vi "Consumer.vi"(8 "error in (no error)":errorcluster, 9 "Data":variant, 10 "Case ID":string, 11 "Tamer in":refnum<class "Tamer.lvclass">) -> (0 "error out":errorcluster, 3 "Tamer out":refnum<class "Tamer.lvclass">)   [LabVIEW 2020, in "Tamer.lvlib" / "Tamer.lvclass"]
uses:
  Tamer.lvclass
  C:/LabVIEW Code/CIRCUS/TALOS/TALOS_PPL.lvlibp/Ancestor/Ancestor/Ancestor.lvclass
  C:/LabVIEW Code/CIRCUS/TALOS/Actor Framework.lvlibp/1abvi3w/vi.lib/ActorFramework/Actor/Actor.lvclass
  C:/LabVIEW Code/CIRCUS/TALOS/TALOS_PPL.lvlibp/Father of all uServices/Father of all uServices/Father of all uServices.lvclass
  Tamer Consumer Case Selector.ctl
  Run Utilities/TypeDefs/Messages/Schedules With Sync Mask Message.ctl
  Run Utilities/Schedule/Schedule.lvclass
  Run Utilities/TypeDefs/Synchronize FPGA Cluster.ctl
  Tamer.lvclass/Tamer.ctl
  TALOS/TALOS_PPL.lvlibp/Ancestor/Ancestor/Infinite Message Selector.ctl
  TALOS/TALOS_PPL.lvlibp/Guardian/Guardian/Requests.ctl
  TALOS/TALOS_PPL.lvlibp/Support VIs/Go-NoGo.ctl
  Run Utilities/TypeDefs/Messages/Append Schedule Message.ctl
  Run Utilities/TypeDefs/Messages/Schedule Message.ctl
  Run Utilities/TypeDefs/DAQ Control.ctl
  Run Utilities/TypeDefs/Messages/Script Checker Message.ctl
  Run Utilities/TypeDefs/Script Checker Result.ctl
  Run Utilities/TypeDefs/Messages/Banana Message.ctl
  Run Utilities/TypeDefs/Return Code.ctl
  Internatl Banana.ctl
  Stop Message.ctl
  TALOS/Actor Framework.lvlibp/1abvi3w/vi.lib/ActorFramework/Message Enqueuer/Message Priority.ctl
  Run Utilities/TypeDefs/Messages/Monkey Status Message.ctl
  Run Utilities/TypeDefs/Monkey Status.ctl
  Monkey Summary.ctl
  Link Chain GUI.ctl
  TALOS/TALOS_PPL.lvlibp/Ancestor/Ancestor/Read ID.vi
  TALOS/TALOS_PPL.lvlibp/Support VIs/Global Constants.vi
  TALOS/TALOS_PPL.lvlibp/Father of all uServices/Father of all uServices/Children Methods/Get GUI Item Value - Variant.vi
  Tamer GV.vi
  TALOS/TALOS_PPL.lvlibp/Father of all uServices/Father of all uServices/Father of all uServices.lvclass
  Run Utilities/Run Utilities.lvlib
  TALOS/TALOS_PPL.lvlibp
  TALOS/TALOS_PPL.lvlibp/Guardian/Guardian/Guardian.lvclass
  TALOS/TALOS_PPL.lvlibp/Ancestor/Ancestor/Ancestor.lvclass
  C:/LabVIEW Code/CIRCUS/CIRCUS uServices et al/Tamer/Tamer.lvclass
  TALOS/TALOS_PPL.lvlibp/Guardian/Guardian Messages/Raise Abort Msg/Raise Abort Msg.lvclass
  TALOS/Actor Framework.lvlibp/1abvi3w/vi.lib/ActorFramework/Actor/Actor.lvclass
  TALOS/Actor Framework.lvlibp/1abvi3w/vi.lib/ActorFramework/Message Enqueuer/Message Enqueuer.lvclass
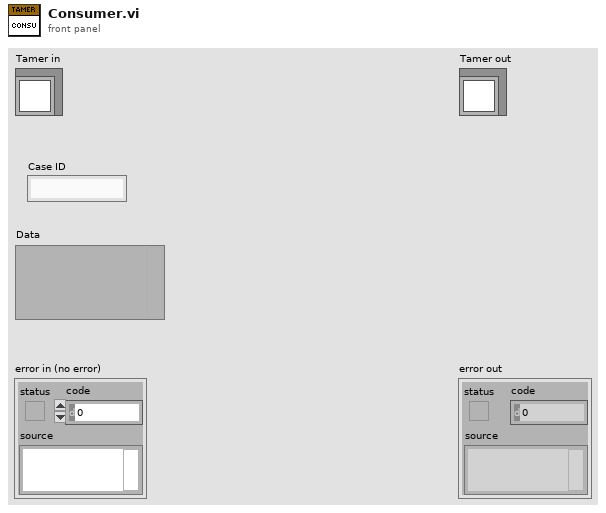
[diagram p1: front panel]
types:
  T1 = typedef "Tamer.lvlib/Tamer.lvclass/Tamer Consumer Case Selector.ctl" = enum16{"New schedule", "Initiate RUN", "Parse Schedules", "Script Checker", "Banana after Quality Check", "Update Crit Lvl", "Propagate Banana", "Reply from Guardian", "Reply from uService", "Timeout of RUN", "uService Replies Check", "Update from Monkey", "Monkey Died", "Reschedule", "Rerun", "Stop DAQ", "Stop Schedule", "Skip Run", "Kill Process", "Update GV", "Append"}
  T2 = typedef "Run Utilities.lvlib/Schedules With Sync Mask Message.ctl" = cluster{"Schedules":refnum<class "Schedule.lvclass">[], "Synchronised":T3[]}
  T3 = typedef "Run Utilities.lvlib/Synchronize FPGA Cluster.ctl" = cluster{"Status":bool, "FPGA Name":string}
  T4 = typedef "TALOS_PPL.lvlibp/Guardian.lvlib/Guardian.lvclass/Requests.ctl" = enum16{"Ready to Launch", "Start RUN", "Stop RUN", "Update DAQ Params", "Update Error Listbox", "Update Run Status", "Update Kasli Log", "Run Stopped with Errors", "Switch uS View"}
  T5 = typedef "TALOS_PPL.lvlibp/Go-NoGo.ctl" = cluster{"ID":string, "Status":bool, "Data":string[], "GUID":string}
  T6 = typedef "Run Utilities.lvlib/Append Schedule Message.ctl" = cluster{"List of FPGAs":set{string}, "Schedules":refnum<class "Schedule.lvclass">[], "To Top?":bool}
  T7 = typedef "Run Utilities.lvlib/Schedule Message.ctl" = cluster{"uS Name":string, "Synchronised":bool, "DAQ Control":T8, "Schedule":refnum<class "Schedule.lvclass">, "Append to top?":bool}
  T8 = typedef "Run Utilities.lvlib/DAQ Control.ctl" = enum16{"On", "Off", "External"}
  T9 = typedef "Run Utilities.lvlib/Script Checker Message.ctl" = cluster{"Monkey ID":string, "Script Checker Result":T10}
  T10 = typedef "Run Utilities.lvlib/Script Checker Result.ctl" = enum16{"Passed", "Failed", "Empty"}
  T11 = typedef "Run Utilities.lvlib/Banana Message.ctl" = cluster{"FPGA Name":string, "Return Code":T12}
  T12 = typedef "Run Utilities.lvlib/Return Code.ctl" = enum16{"All Good", "Retry", "Skip", "Skip All", "ABORT"}
  T13 = typedef "Tamer.lvlib/Tamer.lvclass/Internatl Banana.ctl" = cluster{"Process ID":string, "Return Code":T12}
  T14 = typedef "Tamer.lvlib/Tamer.lvclass/Stop Message.ctl" = cluster{"Gracefully":bool, "Process":string}
  T15 = typedef "Actor Framework.lvlibp/Message Enqueuer.lvclass/Message Priority.ctl" = enum16{"Low", "Normal", "High"}
  T16 = typedef "TALOS_PPL.lvlibp/Ancestor.lvlib/Ancestor.lvclass/Infinite Message Selector.ctl" = enum16{"Start", "Stop", "Check", "Flush (Stop all)", "Init"}
  T17 = typedef "Run Utilities.lvlib/Monkey Status Message.ctl" = cluster{"Monkey ID":string, "Monkey Status":T18, "Scripts left":u32, "ETA":string, "Current Action":string, "Report from previous RUNs":string, "Skipped RUNs":refnum<class "Schedule.lvclass">}
  T18 = typedef "Run Utilities.lvlib/Monkey Status.ctl" = enum16{"Init", "Paused", "Ongoing", "Stopped", "Finished (no errors)", "Finished (with errors)"}
  T19 = typedef "Tamer.lvlib/Tamer.lvclass/Monkey Summary.ctl" = cluster{"Color":u32, "Status":T18, "Continuous":bool, "Scripts left":u32, "Scripts skipped":u32, "ETA":string, "Current Action":string, "Report from previous RUNs":string, "Monkey ID":string, "With DAQ?":bool, "Linked?":T20, "Paused":bool}
  T20 = typedef "Tamer.lvlib/Tamer.lvclass/Link Chain GUI.ctl" = bool
  T21 = typedef "Tamer.lvlib/Tamer.lvclass/Tamer Status.ctl" = cluster{"Monkeys on the Stage":T19[], "All Monkeys Idle":bool}
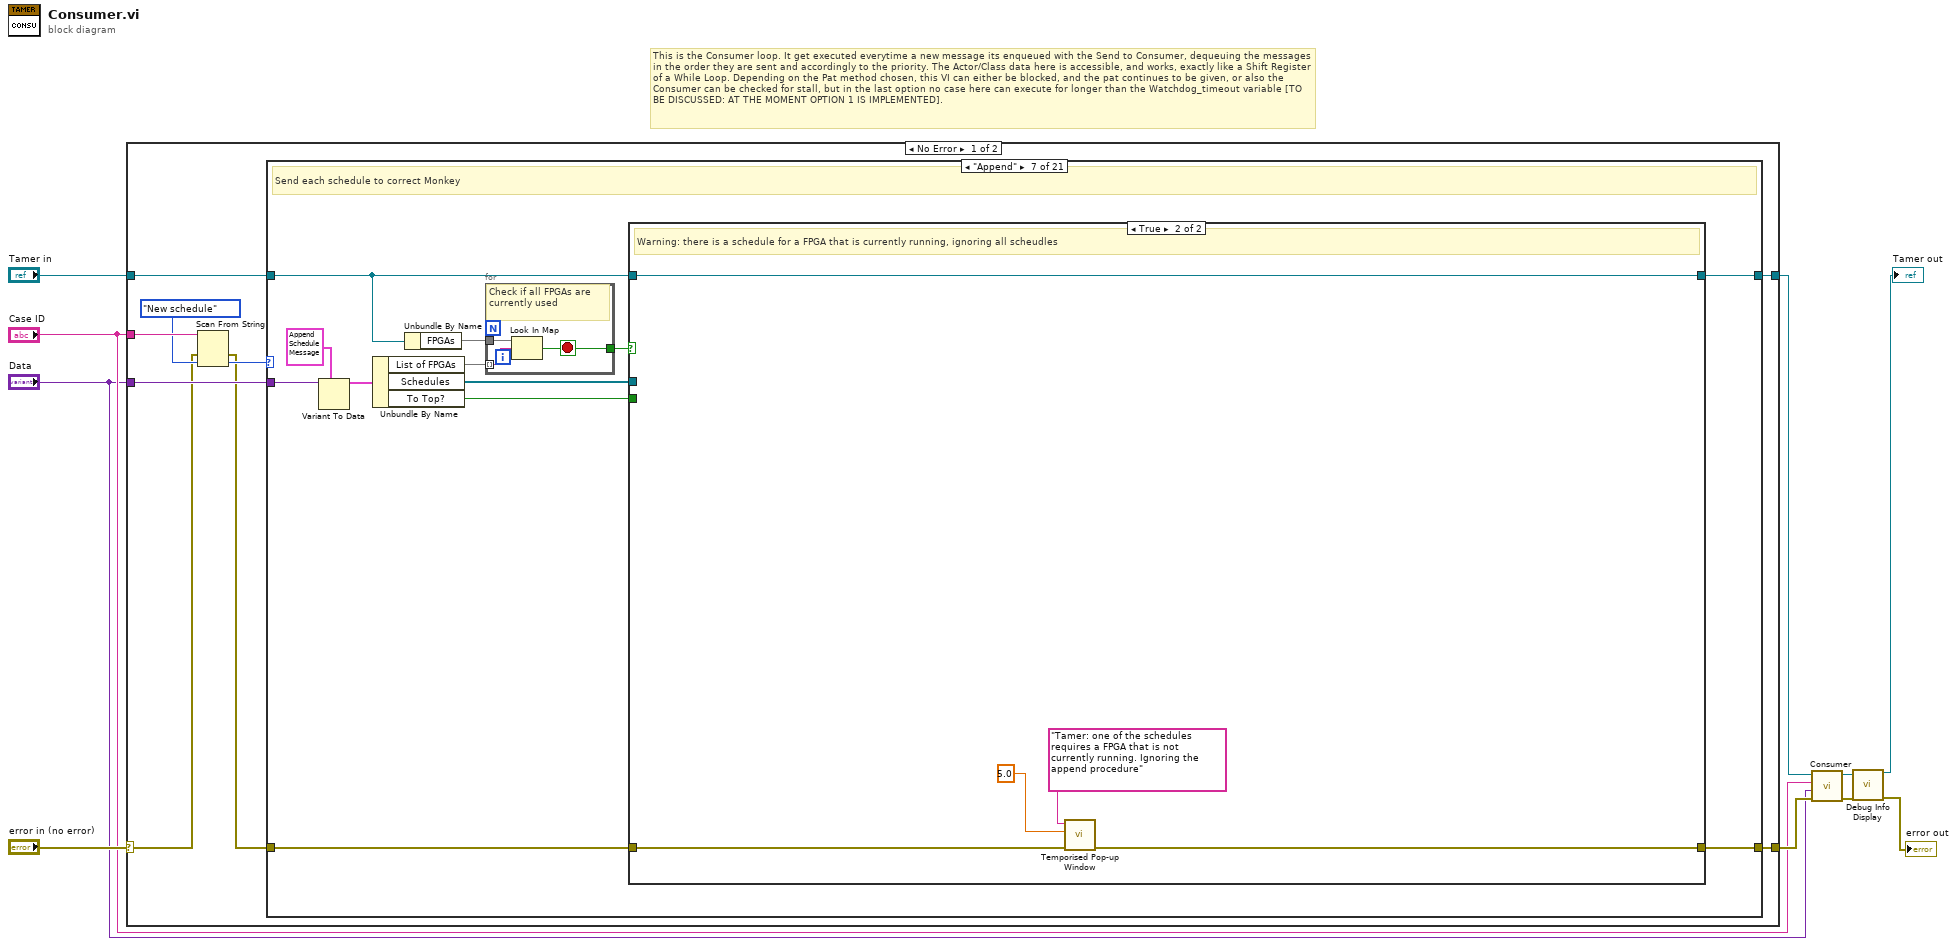
[diagram p0: block diagram]
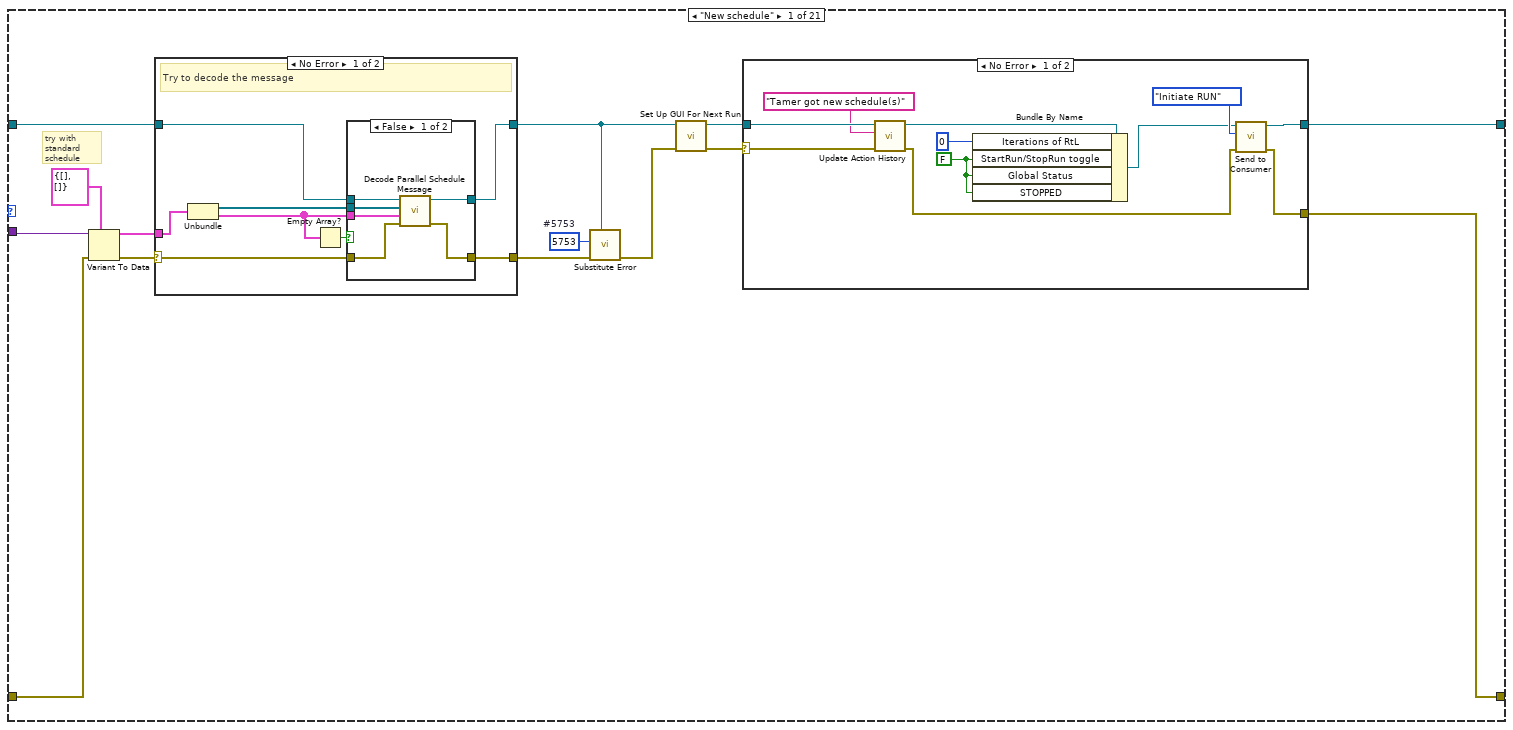
[diagram p2: hidden frame]
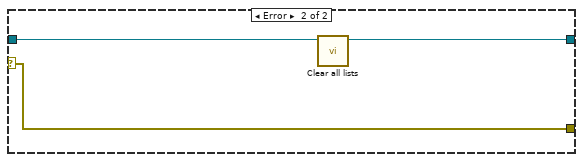
[diagram p3: hidden frame]
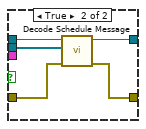
[diagram p4: hidden frame]
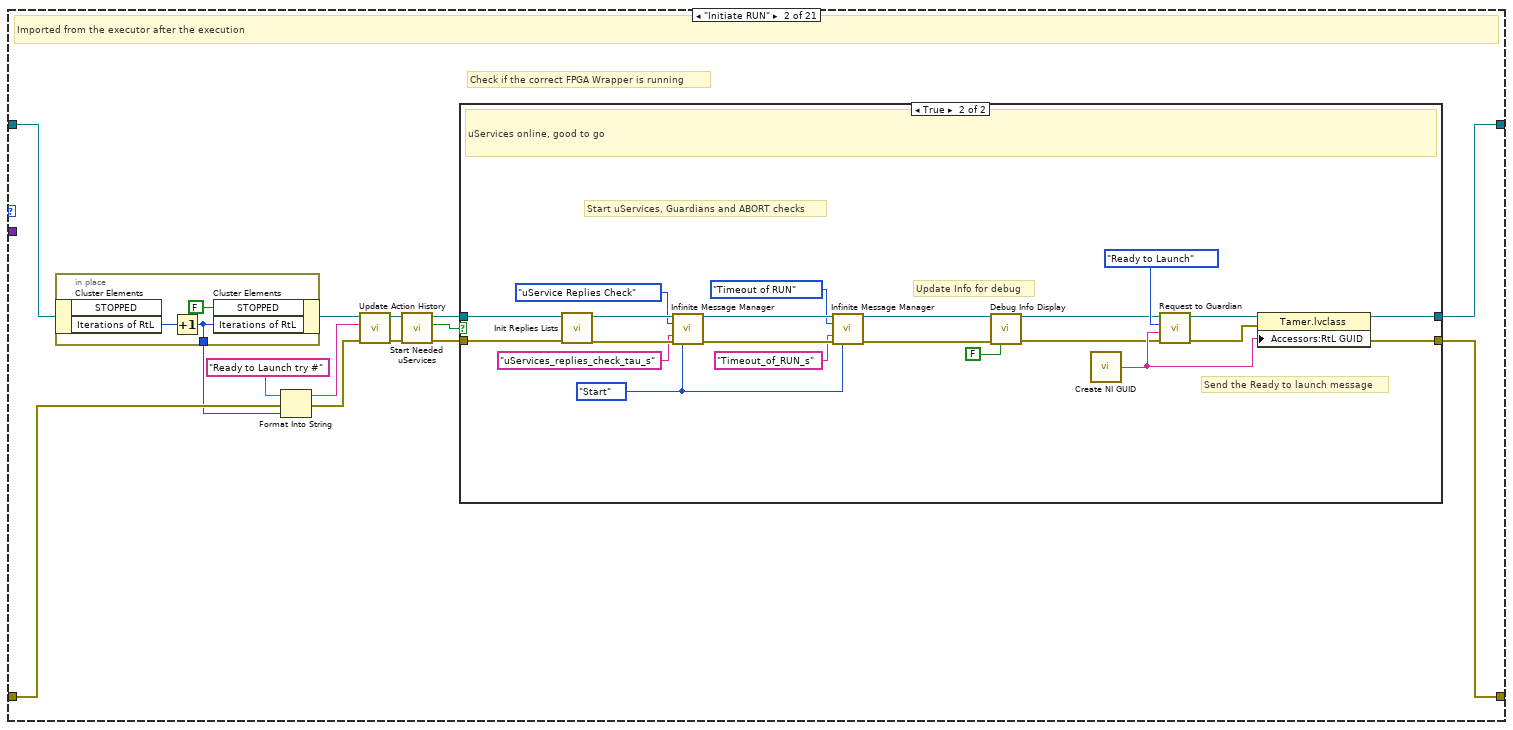
[diagram p6: hidden frame]
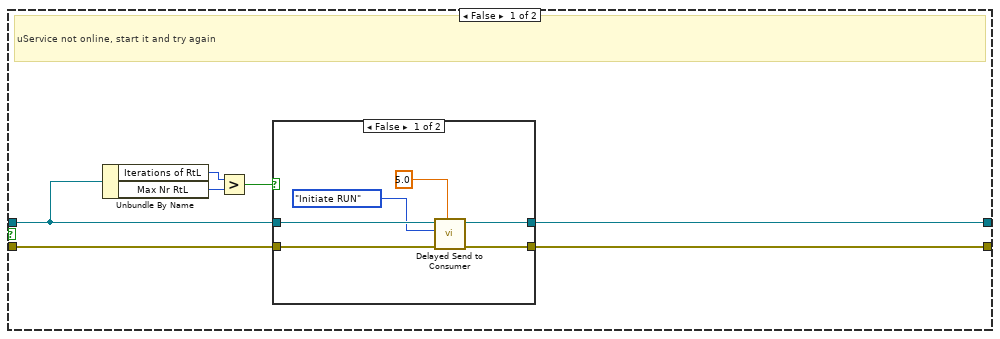
[diagram p7: hidden frame]
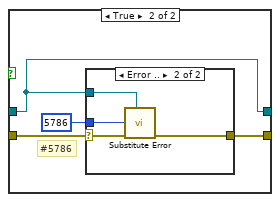
[diagram p8: hidden frame]
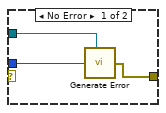
[diagram p9: hidden frame]
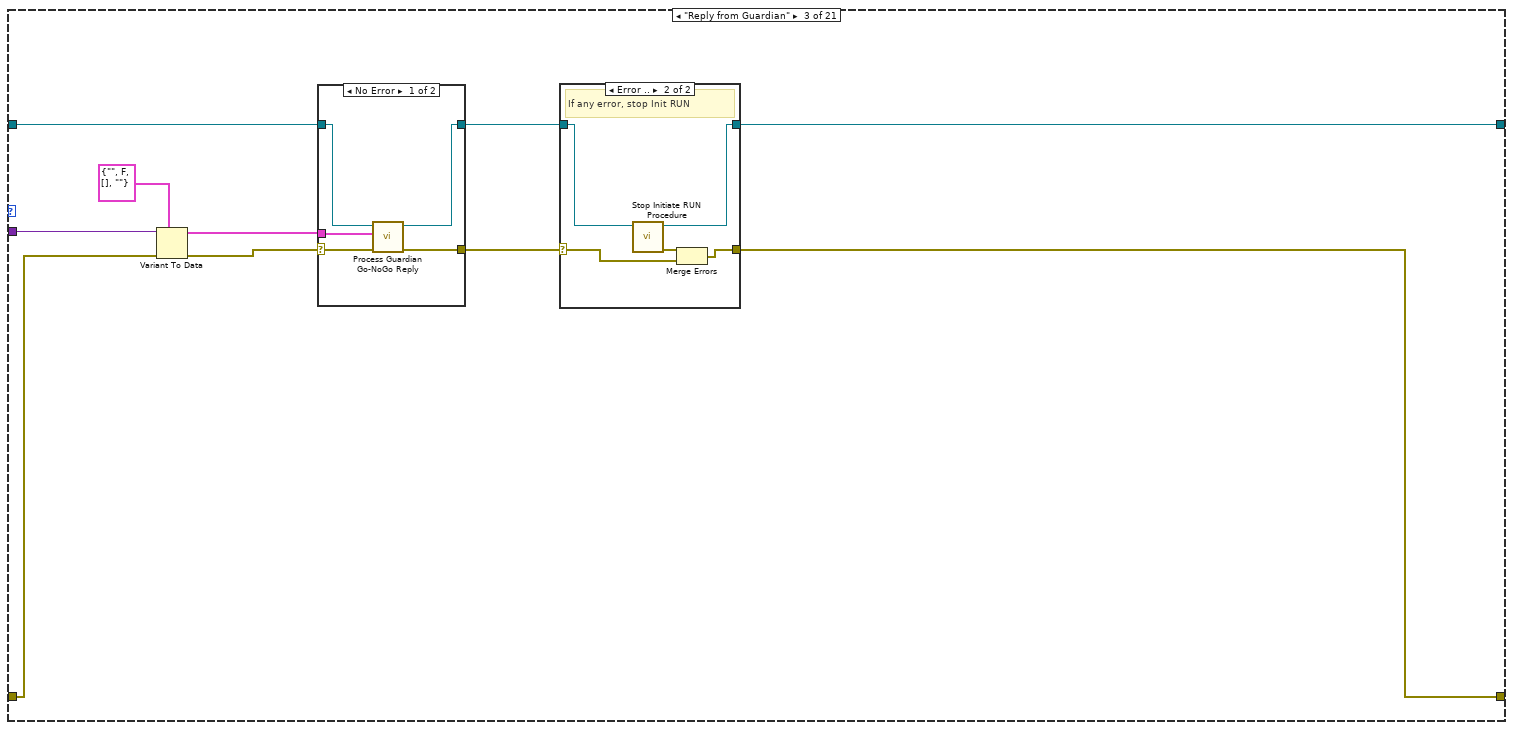
[diagram p10: hidden frame]
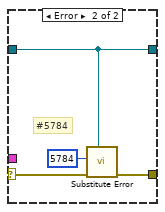
[diagram p12: hidden frame]
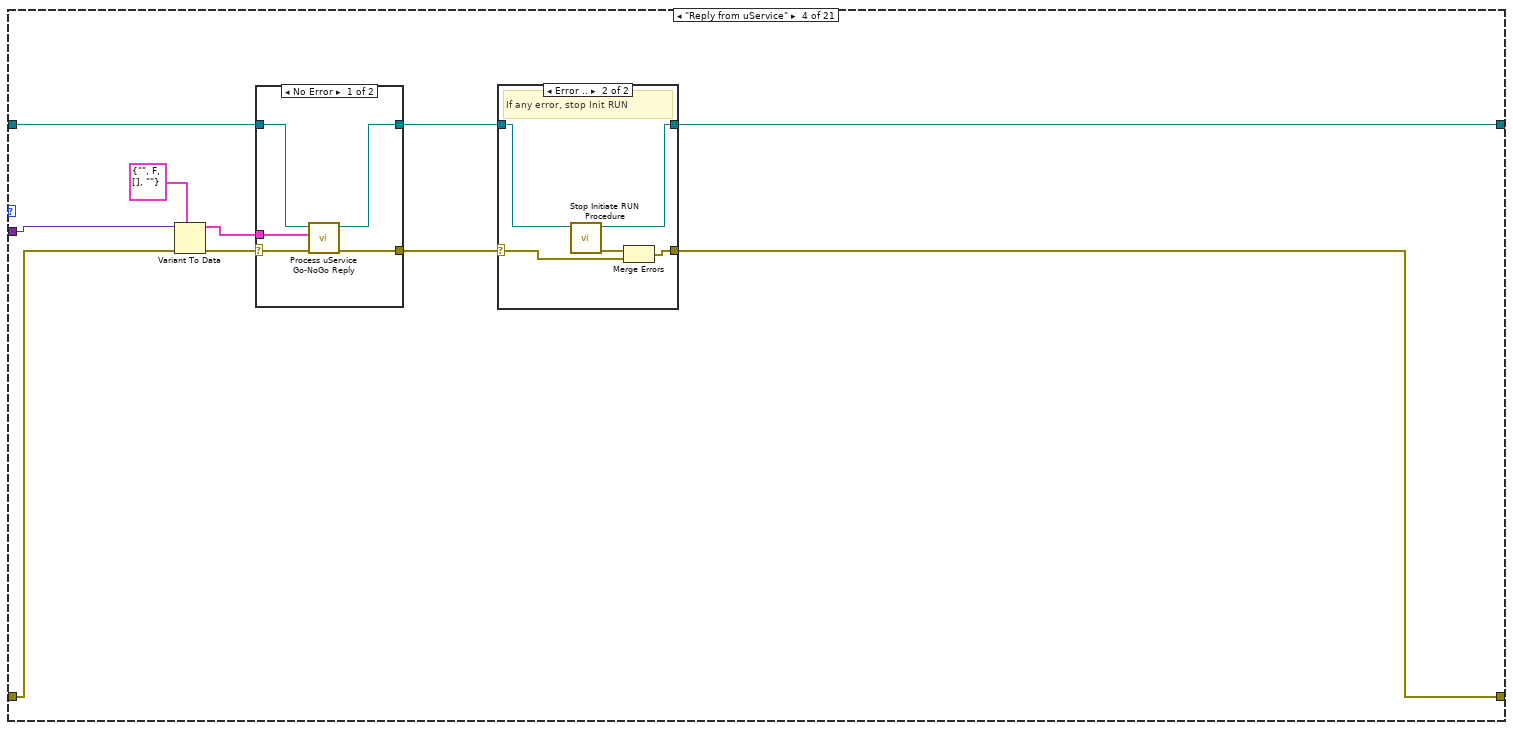
[diagram p13: hidden frame]
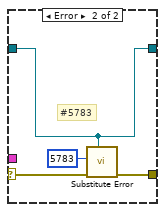
[diagram p15: hidden frame]
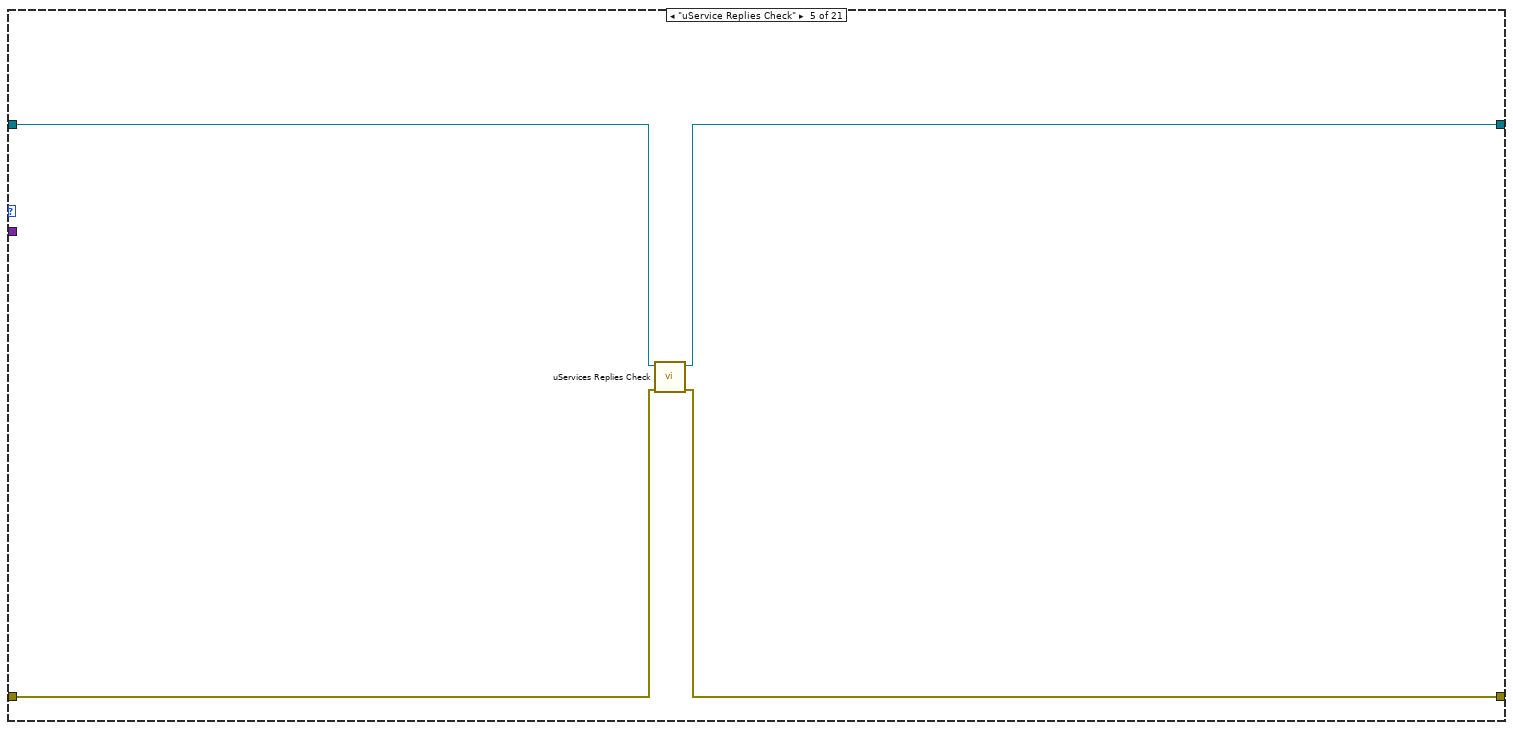
[diagram p16: hidden frame]
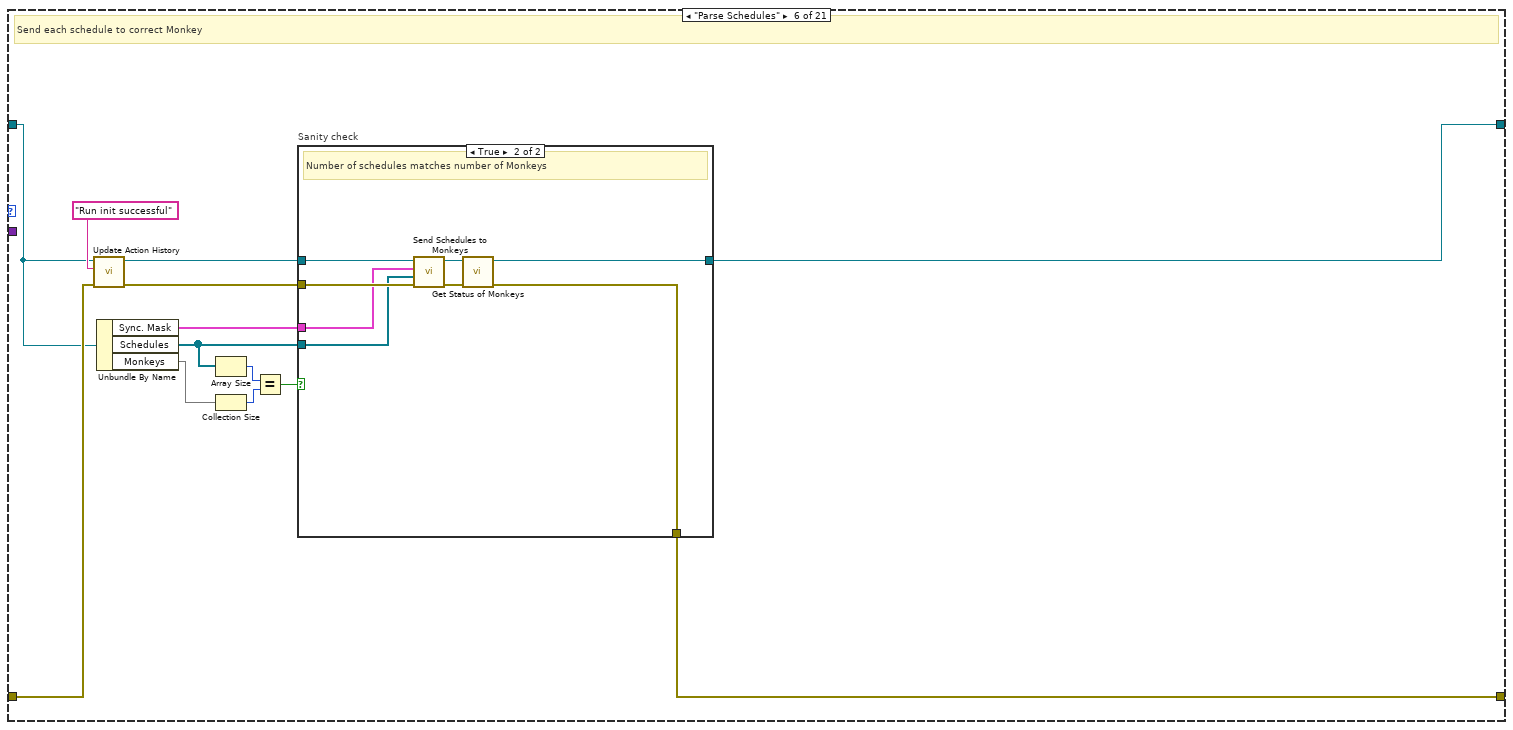
[diagram p17: hidden frame]
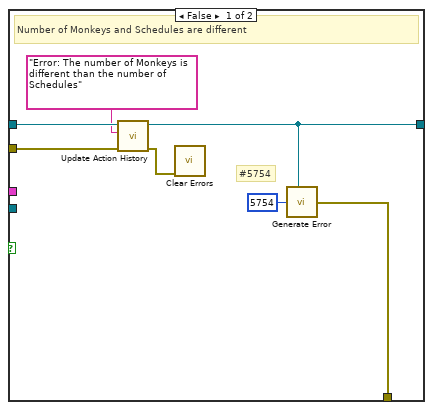
[diagram p18: hidden frame]
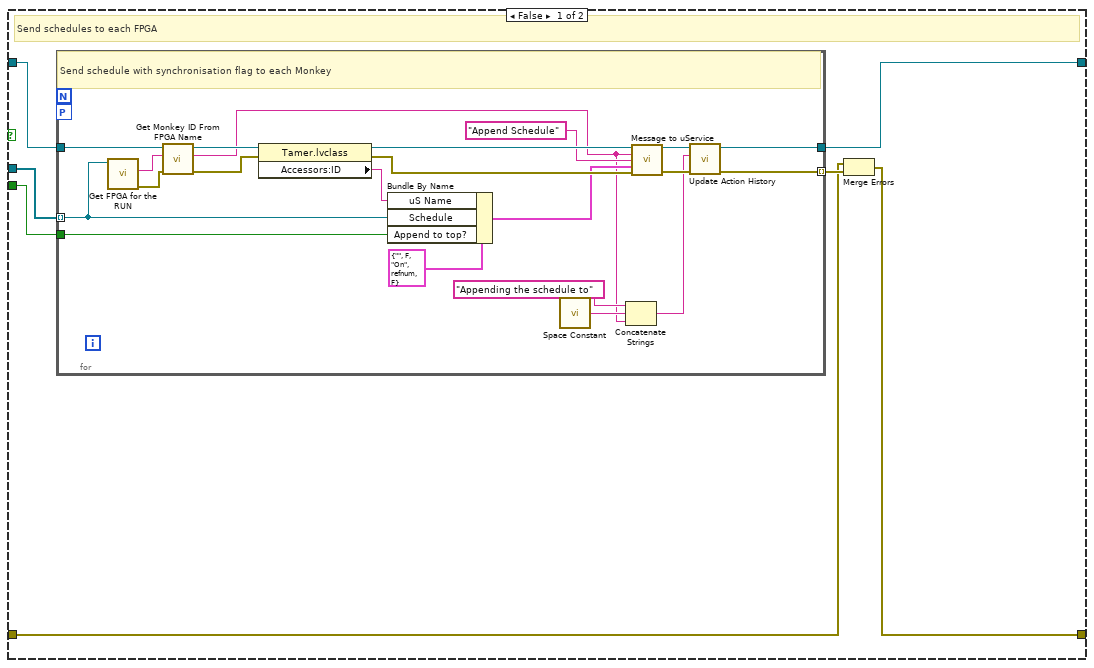
[diagram p19: hidden frame]
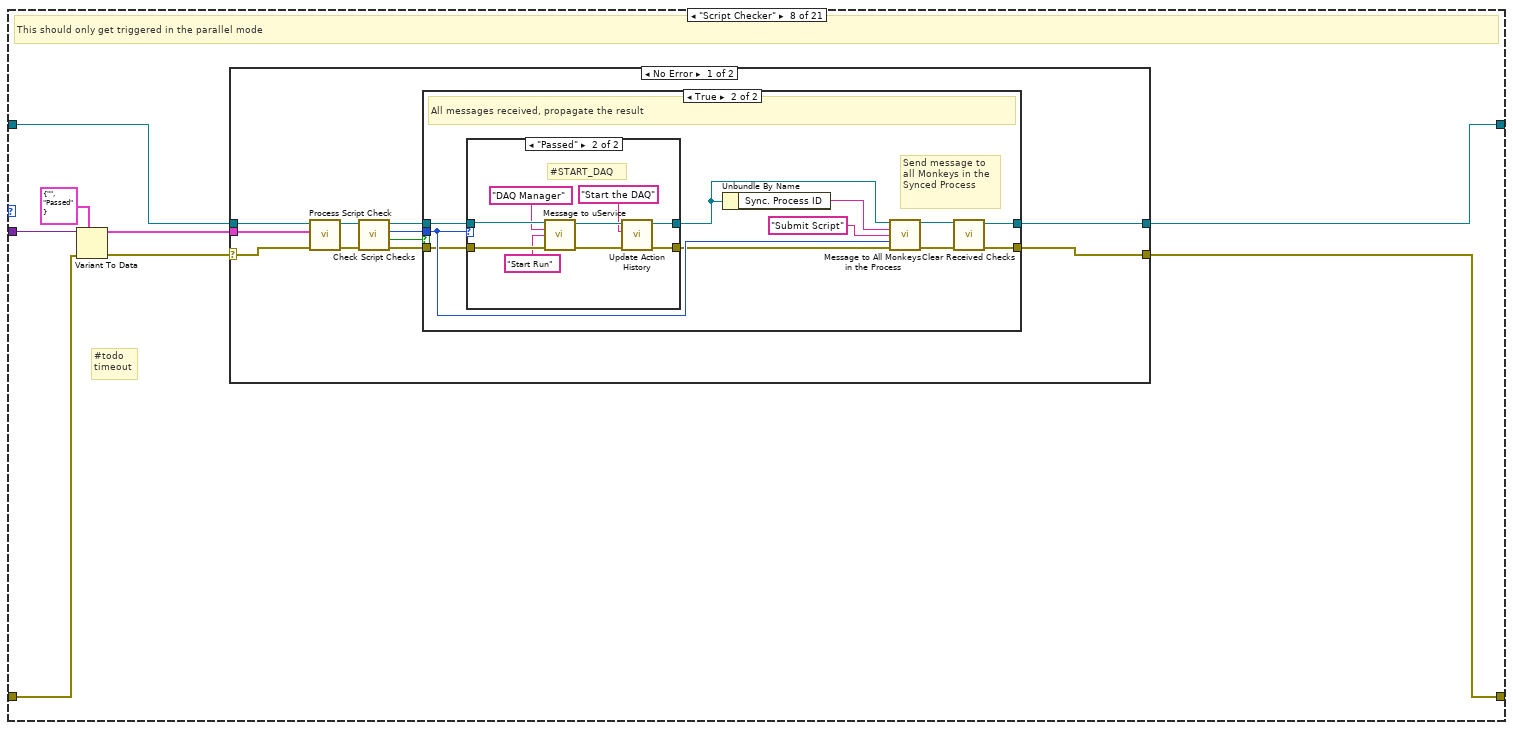
[diagram p20: hidden frame]
diagram:
  # "This is the Consumer loop. It get executed everytime a new message its enqueued with the Send to Consumer, dequeuing the messages in the order they are sent and accordingly to the priority. The Actor/Class data here is accessible, and works, exactly like a Shift Register of a While Loop. Depending on the Pat method chosen, this VI can either be blocked, and the pat continues to be given, or also the Consumer can be checked for stall, but in the last option no case here can execute for longer than the Watchdog_timeout variable [TO BE DISCUSSED: AT THE MOMENT OPTION 1 IS IMPLEMENTED]."
  n1 = case shown="No Error" "error in (no error)" {
    selector: "error in (no error)" -> [w12 w825]
    tunnel: [w18 w826] -> w7
    tunnel: "Tamer in" -> [w19 w826]
    tunnel: [w16 w825] -> w8
    tunnel: "Case ID" -> [w15 _]
    tunnel: "Data" -> [w17 _]
    frame No Error {
      n2 = Scan From String(input string=w15, error in=w12, default 1=Tamer_Consumer_Case_Selector."New schedule" ("Consumer Case Selector")) -> (error out=w11:errorcluster, output 1=w13:T1)  [unwired: 2 in, 2 out]
      n3 = case shown="\"Append\"" w13 {
        tunnel: w19 -> [w29 w69 w137 w163 w184 w191 w219 w266 w311 w378 w384 w403 w469 w485 w553 w593 w628 w677 w753 w817 w823]
        tunnel: [w26 w78 w136 w159 w185 w192 w218 w264 w318 w377 w386 w413 w466 w487 w552 w612 w634 w681 w755 w814 w820] -> w18
        tunnel: w17 -> [w31 _ w135 w162 _ _ w227 w271 w312 _ w390 w415 _ w490 w558 w599 w632 w682 w756 w813 _]
        tunnel: [w25 w77 w133 w160 w186 w198 w216 w265 w317 w375 w385 w412 w467 w486 w551 w611 w636 w680 w754 w815 w819] -> w16
        tunnel: w11 -> [w30 w82 w134 w161 w187 w195 w217 w269 w320 w376 w381 w414 w468 w488 w556 w600 w631 _ w757 w816 w822]
        frame "New schedule" {
          w23 = 5753  # #5753
          # "try with standard schedule"
          n4 = Variant To Data(error in=w30, type=T2 {"Schedules"=[], "Synchronised"=[]} ("Schedule message - parallel"), Variant=w31) -> (data=w32:T2, error out=w33:errorcluster)
          n5 = case shown="No Error" w33 {
            selector: w33 -> [w52 w67]
            tunnel: w32 -> [w48 _]
            tunnel: w29 -> [w54 w68]
            tunnel: [w53 w68] -> w20
            tunnel: [w51 w67] -> w22
            frame No Error {
              # "Try to decode the message"
              n6 = Unbundle(w48) -> ("Schedules"=w55:refnum<class "Schedule.lvclass">[], "Synchronised"=w50:T3[])
              n7 = Empty Array?(array=w50) -> (empty?=w49:bool)
              n8 = case shown="False" w49 {
                tunnel: w55 -> [w57 w66]
                tunnel: w54 -> [w58 w65]
                tunnel: [w59 w64] -> w53
                tunnel: w52 -> [w61 w63]
                tunnel: [w60 w62] -> w51
                tunnel: w50 -> [w56 _]
                frame False {
                  n9 = call-dynamic "Decode Parallel Schedule Message.vi"("error in (no error)"=w61, "Synchronised"=w56, "Schedules"=w57, "Tamer in"=w58) -> ("error out"=w60:errorcluster, "Tamer out"=w59:refnum<class "Tamer.lvclass">)  [unwired: 6 in]
                }
                frame True {
                  n10 = call-dynamic "Decode Schedule Message.vi"("error in (no error)"=w63, "Schedules"=w66, "Tamer in"=w65) -> ("error out"=w62:errorcluster, "Tamer out"=w64:refnum<class "Tamer.lvclass">)  [unwired: 7 in]
                }
              }
            }
            frame Error {
              # "Wrong message type from the Tamer"
            }
          }
          n11 = call "Substitute Error.vi"("LabVIEW Object"=w20, "error in (no error)"=w22, "Error Code"=w23) -> ("error out"=w21:errorcluster)  [unwired: 8 in]
          n12 = call-dynamic "Set Up GUI For Next Run.vi"("error in (no error)"=w21, "Tamer in"=w20) -> ("error out"=w27:errorcluster, "Tamer out"=w28:refnum<class "Tamer.lvclass">)  [unwired: 8 in]
          n13 = case shown="No Error" w27 {
            selector: w27 -> [w39 w47]
            tunnel: [w36 w45] -> w26
            tunnel: w28 -> [w44 w46]
            tunnel: [w34 w47] -> w25
            frame No Error {
              w40 = FALSE ("StartRun/StopRun toggle")
              n14 = call-dynamic "Update Action History.vi"("error in (no error)"=w39, "Action"="Tamer got new schedule(s)", "Tamer in"=w44) -> ("error out"=w35:errorcluster, "Tamer out"=w42:refnum<class "Tamer.lvclass">)  [unwired: 7 in]
              n15 = Bundle By Name(cluster=w42, "Iterations of RtL"=u8 0, "StartRun/StopRun toggle"=w40, "Global Status"=w40, "STOPPED"=w40) -> (w37:refnum<class "Tamer.lvclass">)
              n16 = call "Send to Consumer.vi"("error in (no error)"=w35, "Case ID"=Tamer_Consumer_Case_Selector."Initiate RUN" ("Monkey Consumer Case Selector"), "uService Template in"=w37) -> ("error out"=w34:errorcluster, "uService Template out"=w36:refnum<class "Tamer.lvclass">)  [unwired: 7 in]
            }
            frame Error {
              n17 = call-dynamic "Clear all lists.vi"("Tamer in"=w46) -> ("Tamer out"=w45:refnum<class "Tamer.lvclass">)  [unwired: 9 in, 1 out]
            }
          }
        }
        frame "Initiate RUN" {
          # "Check if the correct FPGA Wrapper is running"
          # "Imported from the executor after the execution"
          n18 = in-place {
            in-place-border: [w83] -> w70
            n19 = in-place-cluster #1(w69) -> ("Iterations of RtL"=w85:u8)  [unwired: 1 out]
            n20 = Increment(x=w85) -> (x+1=w83:u8)
            n21 = in-place-cluster #1("STOPPED"=FALSE, "Iterations of RtL"=w83) -> (w74:refnum<class "Tamer.lvclass">)
          }
          n22 = Format Into String(initial string="Ready to Launch try #", error in=w82, w70) -> (resulting string=w72:string, error out=w71:errorcluster)  [unwired: 1 in]
          n23 = call-dynamic "Update Action History.vi"("error in (no error)"=w71, "Action"=w72, "Tamer in"=w74) -> ("error out"=w75:errorcluster, "Tamer out"=w76:refnum<class "Tamer.lvclass">)  [unwired: 7 in]
          n24 = call-dynamic "Start Needed uServices.vi"("error in (no error)"=w75, "Tamer in"=w76) -> ("error out"=w80:errorcluster, "All online?"=w81:bool, "Tamer out"=w79:refnum<class "Tamer.lvclass">)  [unwired: 7 in]
          n25 = case shown="True" w81 {
            tunnel: w80 -> [w90 w113]
            tunnel: w79 -> [w89 w114]
            tunnel: [w92 w116] -> w78
            tunnel: [w91 w115] -> w77
            frame False {
              # "uService not online, start it and try again"
              n26 = Unbundle By Name(w89) -> ("Iterations of RtL"=w88:u8, "Max Nr RtL"=w87:u8)
              n27 = Greater?(x=w88, y=w87) -> (0:w86:bool)
              n28 = case shown="False" w86 {
                tunnel: [w98 w100] -> w92
                tunnel: [w97 w101] -> w91
                tunnel: w89 -> [w96 w100]
                tunnel: w90 -> [w95 w102]
                frame False {
                  n29 = call "Delayed Send to Consumer.vi"("Seconds (5)"=5.0 ("Delay"), "error in (no error)"=w95, "Case ID"=Tamer_Consumer_Case_Selector."Initiate RUN" ("Tamer Consumer Case Selector"), "Father of all uServices in"=w96) -> ("error out"=w97:errorcluster, "Father of all uServices out"=w98:refnum<class "Tamer.lvclass">)  [unwired: 6 in]
                }
                frame True {
                  # "#5786"
                  n30 = case shown="Error .." w102 {
                    selector: w102 -> [_ w109]
                    tunnel: [w103 w108] -> w101
                    tunnel: w100 -> [w105 w107]
                    tunnel: 5786 -> [w104 w106]
                    frame No Error {
                      n31 = call "Generate Error.vi"("Class"=w105, "Error Code"=w104) -> ("error out"=w103:errorcluster)  [unwired: 5 in]
                    }
                    frame Error {
                      n32 = call "Substitute Error.vi"("LabVIEW Object"=w107, "error in (no error)"=w109, "Error Code"=w106) -> ("error out"=w108:errorcluster)  [unwired: 8 in]
                    }
                  }
                }
              }
            }
            frame True {
              w124 = Infinite_Message_Selector."Start" ("Infinite Message Selector")
              # "Start uServices, Guardians and ABORT checks"
              # "Update Info for debug"
              # "Send the Ready to launch message"
              # "uServices online, good to go"
              n33 = call "Init Replies Lists.vi"("error in (no error)"=w113, "Monkey in"=w114) -> ("error out"=w128:errorcluster, "Monkey out"=w129:refnum<class "Tamer.lvclass">)  [unwired: 8 in]
              n34 = call-dynamic "Infinite Message Manager.vi"("Father of all uServices in"=w129, "Consumer Case Selector"=Tamer_Consumer_Case_Selector."uService Replies Check" ("Monkey Consumer Case Selector"), "Tau parameter"="uServices_replies_check_tau_s" ("SV Name"), "error in (no error)"=w128, "Infinite Message Selector"=w124) -> ("Father of all uServices out"=w126:refnum<class "Tamer.lvclass">, "error out"=w125:errorcluster)  [unwired: 8 in, 1 out]
              n35 = call-dynamic "Infinite Message Manager.vi"("Father of all uServices in"=w126, "Consumer Case Selector"=Tamer_Consumer_Case_Selector."Timeout of RUN" ("Monkey Consumer Case Selector"), "Tau parameter"="Timeout_of_RUN_s" ("SV Name"), "error in (no error)"=w125, "Infinite Message Selector"=w124) -> ("Father of all uServices out"=w120:refnum<class "Tamer.lvclass">, "error out"=w117:errorcluster)  [unwired: 8 in, 1 out]
              n36 = call-dynamic "Debug Info Display.vi"("Tamer in"=w120, "error in (no error)"=w117, "Do not clear"=FALSE) -> ("Tamer out"=w119:refnum<class "Tamer.lvclass">, "error out"=w118:errorcluster)  [unwired: 11 in]
              n37 = call <vilib>:"Create NI GUID.vi"() -> ("NI GUID"=w121:string)
              n38 = call "Request to Guardian.vi"("error in (no error)"=w118, "Data"=w121, "Requests"=Requests."Ready to Launch", "Father of all uServices in"=w119) -> ("error out"=w111:errorcluster, "Father of all uServices out"=w131:refnum<class "Tamer.lvclass">)  [unwired: 6 in]
              n39 = property class="Tamer.lvclass"(reference=w131, error in=w111, "Accessors:RtL GUID"=w121) -> (reference out=w116:refnum<class "Tamer.lvclass">, error out=w115:errorcluster)
            }
          }
        }
        frame "Reply from Guardian" {
          n40 = Variant To Data(error in=w134, type=T5 {"ID"="", "Status"=FALSE, "Data"=[], "GUID"=""} ("Go-NoGo"), Variant=w135) -> (data=w139:T5, error out=w140:errorcluster)
          n41 = case shown="No Error" w140 {
            selector: w140 -> [w153 w156]
            tunnel: [w152 w157] -> w141
            tunnel: w139 -> [w151 _]
            tunnel: w137 -> [w150 w154]
            tunnel: [w149 w154] -> w138
            frame No Error {
              n42 = call "Process Guardian Go-NoGo Reply.vi"("error in (no error)"=w153, "Go-NoGo"=w151, "Tamer in"=w150) -> ("error out"=w152:errorcluster, "Tamer out"=w149:refnum<class "Tamer.lvclass">)  [unwired: 7 in]
            }
            frame Error {
              # "#5784"
              n43 = call "Substitute Error.vi"("LabVIEW Object"=w154, "error in (no error)"=w156, "Error Code"=5784) -> ("error out"=w157:errorcluster)  [unwired: 8 in]
            }
          }
          n44 = case shown="Error .." w141 {
            selector: w141 -> [w143 w145]
            tunnel: [w143 w144] -> w133
            tunnel: [w142 w148] -> w136
            tunnel: w138 -> [w142 w147]
            frame No Error {
              # "All good!"
            }
            frame Error {
              # "If any error, stop Init RUN"
              n45 = call "Stop Initiate RUN Procedure.vi"("Tamer in"=w147) -> ("error out"=w146:errorcluster, "Tamer out"=w148:refnum<class "Tamer.lvclass">)  [unwired: 9 in]
              n46 = Merge Errors(w146, w145) -> (w144:errorcluster)
            }
          }
        }
        frame "Reply from uService" {
          n47 = Variant To Data(error in=w161, type=T5 {"ID"="", "Status"=FALSE, "Data"=[], "GUID"=""} ("Go-NoGo"), Variant=w162) -> (data=w167:T5, error out=w166:errorcluster)
          n48 = case shown="No Error" w166 {
            selector: w166 -> [w178 w182]
            tunnel: w167 -> [w179 _]
            tunnel: [w177 w183] -> w164
            tunnel: [w176 w180] -> w165
            tunnel: w163 -> [w175 w180]
            frame No Error {
              n49 = call "Process uService Go-NoGo Reply.vi"("error in (no error)"=w178, "Go-NoGo"=w179, "Tamer in"=w175) -> ("error out"=w177:errorcluster, "Tamer out"=w176:refnum<class "Tamer.lvclass">)  [unwired: 7 in]
            }
            frame Error {
              # "#5783"
              n50 = call "Substitute Error.vi"("LabVIEW Object"=w180, "error in (no error)"=w182, "Error Code"=5783) -> ("error out"=w183:errorcluster)  [unwired: 8 in]
            }
          }
          n51 = case shown="Error .." w164 {
            selector: w164 -> [w169 w170]
            tunnel: w165 -> [w168 w174]
            tunnel: [w169 w171] -> w160
            tunnel: [w168 w173] -> w159
            frame No Error {
              # "All good!"
            }
            frame Error {
              # "If any error, stop Init RUN"
              n52 = call "Stop Initiate RUN Procedure.vi"("Tamer in"=w174) -> ("error out"=w172:errorcluster, "Tamer out"=w173:refnum<class "Tamer.lvclass">)  [unwired: 9 in]
              n53 = Merge Errors(w172, w170) -> (w171:errorcluster)
            }
          }
        }
        frame "uService Replies Check" {
          n54 = call "uServices Replies Check.vi"("error in (no error)"=w187, "Tamer in"=w184) -> ("error out"=w186:errorcluster, "Tamer out"=w185:refnum<class "Tamer.lvclass">)  [unwired: 8 in]
        }
        frame "Parse Schedules" {
          # "Send each schedule to correct Monkey"
          n55 = call-dynamic "Update Action History.vi"("error in (no error)"=w195, "Action"="Run init successful", "Tamer in"=w191) -> ("error out"=w193:errorcluster, "Tamer out"=w196:refnum<class "Tamer.lvclass">)  [unwired: 7 in]
          n56 = Unbundle By Name(w191) -> ("Sync. Mask"=w200:T3[], "Schedules"=w199:refnum<class "Schedule.lvclass">[], "Monkeys"=w189:map{string, string[]})
          n57 = Array Size(array=w199) -> (size(s)=w190:i32)
          n58 = Collection Size(1:w189) -> (0:w188:i32)
          n59 = Equal?(x=w190, y=w188) -> (x = y?=w197:bool)
          n60 = case "Sanity check" shown="True" w197 {
            tunnel: w200 -> [_ w212]
            tunnel: w196 -> [w205 w214]
            tunnel: w199 -> [_ w213]
            tunnel: [w206 w208] -> w198
            tunnel: w193 -> [w204 w215]
            tunnel: [w201 w210] -> w192
            frame False {
              # "#5754"
              # "Number of Monkeys and Schedules are different"
              n61 = call-dynamic "Update Action History.vi"("error in (no error)"=w204, "Action"="Error: The number of Monkeys is different than the number of Schedules", "Tamer in"=w205) -> ("error out"=w202:errorcluster, "Tamer out"=w201:refnum<class "Tamer.lvclass">)  [unwired: 7 in]
              n62 = call <vilib>:"Clear Errors.vi"("error in (no error)"=w202) -> ()  [unwired: 5 in, 2 out]
              n63 = call "Generate Error.vi"("Class"=w201, "Error Code"=5754) -> ("error out"=w206:errorcluster)  [unwired: 5 in]
            }
            frame True {
              # "Number of schedules matches number of Monkeys"
              n64 = call "Send Schedules to Monkeys.vi"("error in (no error)"=w215, "Schedules"=w213, "Sync. Mask"=w212, "Tamer in"=w214) -> ("error out"=w209:errorcluster, "Tamer out"=w211:refnum<class "Tamer.lvclass">)  [unwired: 6 in]
              n65 = call-dynamic "Get Status of Monkeys.vi"("error in (no error)"=w209, "Tamer in"=w211) -> ("error out"=w208:errorcluster, "Tamer out"=w210:refnum<class "Tamer.lvclass">)  [unwired: 7 in, 1 out]
            }
          }
        }
        frame "Append" {
          # "Send each schedule to correct Monkey"
          n66 = Variant To Data(type=T6 {"List of FPGAs"={}, "Schedules"=[], "To Top?"=FALSE} ("Schedule message"), Variant=w227) -> (data=w225:T6)  [unwired: 1 in, 1 out]
          n67 = Unbundle By Name(w225) -> ("List of FPGAs"=w224:set{string}, "Schedules"=w221:refnum<class "Schedule.lvclass">[], "To Top?"=w220:bool)
          n68 = Unbundle By Name(w219) -> ("FPGAs"=w223:map{string, string})
          n69 = for {
            tunnel: w224 -> [w262] mode=indexing
            tunnel: w223 -> [w263]
            tunnel: [w261] -> w222
            stop <- w261 stop-if-true
            # "Check if all FPGAs are currently used"
            n70 = Look In Map(map=w263, key=w262) -> (key not found?=w261:bool)  [unwired: 1 in, 1 out]
          }
          n71 = case shown="True" w222 {
            tunnel: w221 -> [w232 _]
            tunnel: w220 -> [w231 _]
            tunnel: w219 -> [w234 w260]
            tunnel: [w233 w260] -> w218
            tunnel: w217 -> [w228 w257]
            tunnel: [w229 w256] -> w216
            frame False {
              # "Send schedules to each FPGA"
              n72 = for {
                tunnel: w234 -> [w244]
                tunnel: w232 -> [w238] mode=indexing
                tunnel: [w236] -> w230 mode=indexing
                tunnel: [w237] -> w233
                workers-P: _ -> [_]
                tunnel: w231 -> [w235]
                # "Send schedule with synchronisation flag to each Monkey"
                n73 = call-dynamic "Get FPGA for the RUN.vi"("Schedule in"=w238) -> ("error out"=w241:errorcluster, "FPGA Name"=w242:string)  [unwired: 8 in, 1 out]
                n74 = call-dynamic "Get Monkey ID From FPGA Name.vi"("error in (no error)"=w241, "FPGA Name"=w242, "Tamer in"=w244) -> ("error out"=w240:errorcluster, "Monkey ID"=w239:string, "Tamer out"=w243:refnum<class "Tamer.lvclass">)  [unwired: 6 in]
                n75 = property class="Tamer.lvclass"(reference=w243, error in=w240) -> (reference out=w252:refnum<class "Tamer.lvclass">, error out=w255:errorcluster, "Accessors:ID"=w251:string)
                n76 = Bundle By Name(cluster=T7 {"uS Name"="", "Synchronised"=FALSE, "DAQ Control"=enum."On", "Schedule"=refnum, "Append to top?"=FALSE} ("Monkey Schedule Message"), "uS Name"=w251, "Schedule"=w238, "Append to top?"=w235) -> (w254:T7)
                n77 = call <vilib>:"Space Constant.vi"() -> ("String"=w246:string)
                n78 = Concatenate Strings("Appending the schedule to" ("string"), w246, w239) -> (w248:string)
                n79 = call "Message to uService.vi"("Father of all uServices in"=w252, "uService ID"=w239, "Message"="Append Schedule", "Data"=w254, "error in (no error)"=w255) -> ("Father of all uServices out"=w250:refnum<class "Tamer.lvclass">, "error out"=w249:errorcluster)  [unwired: 9 in]
                n80 = call-dynamic "Update Action History.vi"("error in (no error)"=w249, "Action"=w248, "Tamer in"=w250) -> ("error out"=w236:errorcluster, "Tamer out"=w237:refnum<class "Tamer.lvclass">)  [unwired: 7 in]
              }
              n81 = Merge Errors(w228, w230) -> (w229:errorcluster)
            }
            frame True {
              # "Warning: there is a schedule for a FPGA that is currently running, ignoring all scheudles"
              n82 = call "Temporised Pop-up Window.vi"("error in (no error)"=w257, "Timeout"=5.0, "Text"="Tamer: one of the schedules requires a FPGA that is not currently running. Ignoring the append procedure") -> ("error out"=w256:errorcluster)  [unwired: 8 in]
            }
          }
        }
        frame "Script Checker" {
          # "#todo\ntimeout"
          # "This should only get triggered in the parallel mode"
          n83 = Variant To Data(error in=w269, type=T9 {"Monkey ID"="", "Script Checker Result"=enum."Passed"} ("Message"), Variant=w271) -> (data=w267:T9, error out=w268:errorcluster)
          n84 = case shown="No Error" w268 {
            selector: w268 -> [w282 w310]
            tunnel: w267 -> [w273 _]
            tunnel: w266 -> [w274 w308]
            tunnel: [w272 w309] -> w265
            tunnel: [w275 w308] -> w264
            frame No Error {
              n85 = call-dynamic "Process Script Check.vi"("error in (no error)"=w282, "Message"=w273, "Tamer in"=w274) -> ("error out"=w280:errorcluster, "Tamer out"=w281:refnum<class "Tamer.lvclass">)  [unwired: 7 in]
              n86 = call-dynamic "Check Script Checks.vi"("error in (no error)"=w280, "Tamer in"=w281) -> ("error out"=w278:errorcluster, "Send Result?"=w279:bool, "Script Checker Result"=w277:T10, "Tamer out"=w276:refnum<class "Tamer.lvclass">)  [unwired: 6 in]
              n87 = case shown="True" w279 {
                tunnel: w278 -> [w283 w288]
                tunnel: w277 -> [_ w293]
                tunnel: w276 -> [w284 w287]
                tunnel: [w283 w290] -> w272
                tunnel: [w284 w289] -> w275
                frame False {
                  # "Waiting for some responses"
                }
                frame True {
                  # "Send message to all Monkeys in the Synced Process"
                  # "All messages received, propagate the result"
                  n88 = case shown="\"Passed\"" w293 {
                    tunnel: w287 -> [w297 w300]
                    tunnel: w288 -> [w296 w303]
                    tunnel: [w296 w302] -> w285
                    tunnel: [w297 w301] -> w286
                    frame Default {
                    }
                    frame "Passed" {
                      # "#START_DAQ"
                      n89 = call "Message to uService.vi"("Father of all uServices in"=w300, "uService ID"="DAQ Manager", "Message"="Start Run", "error in (no error)"=w303) -> ("Father of all uServices out"=w305:refnum<class "Tamer.lvclass">, "error out"=w306:errorcluster)  [unwired: 10 in]
                      n90 = call-dynamic "Update Action History.vi"("error in (no error)"=w306, "Action"="Start the DAQ", "Tamer in"=w305) -> ("error out"=w302:errorcluster, "Tamer out"=w301:refnum<class "Tamer.lvclass">)  [unwired: 7 in]
                    }
                  }
                  n91 = Unbundle By Name(w286) -> ("Sync. Process ID"=w294:string)
                  n92 = call-dynamic "Message to All Monkeys in the Process.vi"("Tamer in"=w286, "Process ID"=w294, "Message"="Submit Script", "Data"=w293, "error in (no error)"=w285) -> ("Tamer out"=w292:refnum<class "Tamer.lvclass">, "error out"=w291:errorcluster)  [unwired: 9 in]
                  n93 = call-dynamic "Clear Received Checks.vi"("error in (no error)"=w291, "Tamer in"=w292) -> ("error out"=w290:errorcluster, "Tamer out"=w289:refnum<class "Tamer.lvclass">)  [unwired: 8 in]
                }
              }
            }
            frame Error {
              # "#5207"
              n94 = call "Substitute Error.vi"("LabVIEW Object"=w308, "error in (no error)"=w310, "Error Code"=5207) -> ("error out"=w309:errorcluster)  [unwired: 8 in]
            }
          }
        }
        frame "Banana after Quality Check" {
          # "This case is needed to avoid the race condition of an error getting enqueued immediately after the Run is finished: the Monkey would then skip the Criticality Level associated to that error (and, by the way, using it in the subsequent Run). In this way, the \"What to do next\" will be enqued after any - reasonably - possible \"Error Criticality\" message from the Error Manager."
          n95 = Variant To Data(error in=w320, type=T11 {"FPGA Name"="", "Return Code"=enum."All Good"} ("Cluster"), Variant=w312) -> (data=w315:T11, error out=w316:errorcluster)
          n96 = case shown="Error .." w316 {
            selector: w316 -> [w321 _]
            tunnel: w315 -> [w322 _]
            tunnel: [w322 w331] -> w314
            tunnel: [w321 w327] -> w313
            tunnel: w312 -> [_ w330]
            tunnel: w311 -> [_ w326]
            frame No Error {
            }
            frame Error {
              n97 = Variant To Data(type="", Variant=w330) -> (data=w325:string, error out=w328:errorcluster)  [unwired: 1 in]
              n98 = call-dynamic "Get FPGA Name From Monkey ID.vi"("error in (no error)"=w328, "Monkey ID"=w325, "Tamer in"=w326) -> ("error out"=w327:errorcluster, "FPGA Name"=w324:string)  [unwired: 6 in, 1 out]
              n99 = Bundle By Name(cluster=T11 {"FPGA Name"="", "Return Code"=enum."All Good"} ("Cluster"), "Return Code"=Return_Code."Skip", "FPGA Name"=w324) -> (w331:T11)
            }
          }
          n100 = case shown="No Error" w313 {
            selector: w313 -> [w340 w369]
            tunnel: [w336 w373] -> w318
            tunnel: [w333 w372] -> w317
            tunnel: w311 -> [w335 w373]
            tunnel: w314 -> [w334 _]
            frame No Error {
              n101 = call-dynamic "Process Banana Message.vi"("error in (no error)"=w340, "Message"=w334, "Tamer in"=w335) -> ("error out"=w341:errorcluster, "Propagate Banana?"=w339:bool, "Internal Banana"=w337:T13, "Tamer out"=w338:refnum<class "Tamer.lvclass">)  [unwired: 5 in]
              n102 = case shown="True" w339 {
                tunnel: w338 -> [w343 w353]
                tunnel: w341 -> [w342 w354]
                tunnel: w337 -> [_ w344]
                tunnel: [w343 w348] -> w336
                tunnel: [w342 w346] -> w333
                frame False {
                  # "Do not propagate Banana (maybe not all Monkeys finished, or there was ABORT)"
                }
                frame True {
                  # "avoid enqueuing a new script before the previous one has finished"
                  # "Let's Propagate with a delay"
                  n103 = Unbundle By Name(w353) -> ("Sync. Process ID"=w352:string)
                  n104 = Unbundle By Name(w344) -> ("Process ID"=w351:string)
                  n105 = Equal?(x=w352, y=w351) -> (x = y?=w350:bool)
                  n106 = case shown="True" w350 {
                    tunnel: w354 -> [w358 w367]
                    tunnel: [w361 w368] -> w349
                    tunnel: [w356 w367] -> w347
                    tunnel: w353 -> [w360 w368]
                    tunnel: [w362 1.0] -> w355
                    frame True {
                      # "#STOP_DAQ"
                      # "In synchronised we need to stop DAQ"
                      n107 = call "Send to Consumer.vi"("error in (no error)"=w358, "Case ID"=Tamer_Consumer_Case_Selector."Stop DAQ" ("Consumer Case Selector"), "uService Template in"=w360) -> ("error out"=w357:errorcluster, "uService Template out"=w361:refnum<class "Tamer.lvclass">)  [unwired: 7 in]
                      n108 = call "TALOS Config Param.vi"("error in (no error)"=w357, "Parameter Name"="Stop_DAQ_Delay_s") -> ("error out"=w356:errorcluster, "Output"=w364:string)  [unwired: 8 in]
                      n109 = Fract/Exp String To Number(string=w364, default (0 dbl)=10.0 ("default (0 DBL)")) -> (number=w362:dbl)  [unwired: 2 in, 1 out]
                    }
                    frame False {
                      # "Not synchronised, just send it"
                    }
                  }
                  n110 = call "Delayed Send to Consumer.vi"("Seconds (5)"=w355, "error in (no error)"=w347, "Data"=w344, "Case ID"=Tamer_Consumer_Case_Selector."Propagate Banana" ("Consumer Case Selector"), "Father of all uServices in"=w349) -> ("error out"=w346:errorcluster, "Father of all uServices out"=w348:refnum<class "Tamer.lvclass">)  [unwired: 5 in]
                }
              }
            }
            frame Error {
              # "#5207"
              n111 = call "Substitute Error.vi"("LabVIEW Object"=w373, "error in (no error)"=w369, "Error Code"=5207, "Optional String"="Wrong banana message!") -> ("error out"=w372:errorcluster)  [unwired: 7 in]
            }
          }
        }
        frame "Stop DAQ" {
          # "#STOP_DAQ"
          n112 = call "Message to uService.vi"("Father of all uServices in"=w378, "uService ID"="DAQ Manager", "Message"="Stop Run", "error in (no error)"=w376) -> ("Father of all uServices out"=w377:refnum<class "Tamer.lvclass">, "error out"=w375:errorcluster)  [unwired: 10 in]
        }
        frame "Propagate Banana" {
          # "By default, I mean"
          # "#Stop or ABORT?"
          # "Send Processed Banana to each Monkey that needs to receive it"
          n113 = call-dynamic "Update Action History.vi"("error in (no error)"=w381, "Action"="Propagate Banana", "Tamer in"=w384) -> ("error out"=w382:errorcluster, "Tamer out"=w383:refnum<class "Tamer.lvclass">)  [unwired: 7 in]
          n114 = Variant To Data(error in=w382, type=T13 {"Process ID"="", "Return Code"=enum."All Good"} ("Internal Banana"), Variant=w390) -> (data=w388:T13, error out=w387:errorcluster)
          n115 = case shown="No Error" w387 {
            selector: w387 -> [w395 w402]
            tunnel: w388 -> [w398 _]
            tunnel: [w394 w400] -> w386
            tunnel: [w393 w401] -> w385
            tunnel: w383 -> [w391 w400]
            frame No Error {
              n116 = Unbundle By Name(w398) -> ("Process ID"=w397:string, "Return Code"=w396:T12)
              n117 = call-dynamic "Message to All Monkeys in the Process.vi"("Tamer in"=w391, "Process ID"=w397, "Message"="B4N4N4", "Data"=w396, "error in (no error)"=w395) -> ("Tamer out"=w394:refnum<class "Tamer.lvclass">, "error out"=w393:errorcluster)  [unwired: 9 in]
            }
            frame Error {
              # "#5207"
              n118 = call "Substitute Error.vi"("LabVIEW Object"=w400, "error in (no error)"=w402, "Error Code"=5207) -> ("error out"=w401:errorcluster)  [unwired: 8 in]
            }
          }
        }
        frame "Update Crit Lvl" {
          # "Volpe: it is correct to forward the criticality level to each Monkey and let them handle it, because if they are running async, they need to independently choose what to do"
          # "If there was an error in variant to data, it means that the variant was empty: no specific error was provided. Ignore that error"
          # "Send Criticality level to every Running Monkey. so it knows"
          n119 = Variant To Data(error in=w414, type=u8 0, Variant=w415) -> (data=w410:u8, error out=w411:errorcluster)
          n120 = global read "Global Constants.vi" "ABORT Crt Lvl"() -> (w406:u8)
          n121 = case shown="No Error" w411 {
            selector: w411 -> [w459 w464]
            tunnel: w410 -> [w460 _]
            tunnel: [w460 w461] -> w409
            tunnel: [w459 w463] -> w408
            tunnel: w406 -> [_ w462]
            frame No Error {
            }
            frame Error {
              n122 = call <vilib>:"Clear Errors.vi"("error in (no error)"=w464) -> ("error out"=w463:errorcluster)  [unwired: 5 in, 1 out]
              n123 = Decrement(x=w462) -> (x-1=w461:u8)
            }
          }
          n124 = case shown="No Error" w408 {
            selector: w408 -> [w444 w458]
            tunnel: w409 -> [w447 _]
            tunnel: [w443 w457] -> w405
            tunnel: [w442 w455] -> w404
            tunnel: w406 -> [w441 w455]
            tunnel: w403 -> [w440 w454]
            frame No Error {
              n125 = In Range and Coerce(upper limit=w441, x=w447, lower limit=u8 0) -> (In Range?=w445:bool)  [unwired: 1 out]
              n126 = case shown="False" w445 {
                tunnel: w447 -> [_ w453]
                tunnel: w444 -> [_ w452]
                tunnel: [w451 w452] -> w443
                tunnel: [w449 w453] -> w442
                tunnel: w441 -> [w449 _]
                tunnel: w440 -> [w448 _]
                frame False {
                  # "#5788"
                  n127 = call "Generate Error.vi"("Class"=w448, "Error Code"=5788) -> ("error out"=w451:errorcluster)  [unwired: 5 in]
                }
                frame True {
                  # "All good!"
                }
              }
            }
            frame Error {
              # "#5788"
              n128 = call "Substitute Error.vi"("LabVIEW Object"=w454, "error in (no error)"=w458, "Error Code"=5788) -> ("error out"=w457:errorcluster)  [unwired: 8 in]
            }
          }
          n129 = case shown="4" w404 {
            selector: w404 -> [w416 _ _]
            tunnel: w403 -> [w420 w431 w436]
            tunnel: w405 -> [w419 w429 w433]
            tunnel: [w417 w423 w438] -> w413
            tunnel: [w418 w428 w432] -> w412
            frame Default {
              n130 = call-dynamic "Send Error Criticality.vi"("error in (no error)"=w419, "Crit. Level"=w416, "Tamer in"=w420) -> ("error out"=w418:errorcluster, "Tamer out"=w417:refnum<class "Tamer.lvclass">)  [unwired: 5 in]
            }
            frame 3 {
              # "To stop gracefully all the running processes"
              n131 = call "Send to Consumer.vi"("Data"=T14 {"Gracefully"=TRUE, "Process"="ALL"} ("cluster"), "Case ID"=Tamer_Consumer_Case_Selector."Stop Schedule" ("Monkey Consumer Case Selector"), "uService Template in"=w431) -> ("error out"=w424:errorcluster, "uService Template out"=w425:refnum<class "Tamer.lvclass">)  [unwired: 7 in]
              n132 = call "Request to Guardian.vi"("error in (no error)"=w424, "Data"=FALSE, "Requests"=Requests."Run Stopped with Errors", "Father of all uServices in"=w425) -> ("error out"=w422:errorcluster, "Father of all uServices out"=w423:refnum<class "Tamer.lvclass">)  [unwired: 6 in]
              n133 = Merge Errors(w422, w429) -> (w428:errorcluster)
            }
            frame 4 {
              # "Let safe mode do the work"
              n134 = call "Read Caller Enqueuer.vi"("Actor"=w436) -> ("Caller Enqueuer"=w435:refnum<class "Message Enqueuer.lvclass">)  [unwired: 10 in]
              n135 = call "Send Raise Abort.vi"("Message Priority (Normal)"=Message_Priority."High", "error in (no error)"=w433, "Message Enqueuer"=w435) -> ("error out"=w432:errorcluster)  [unwired: 7 in, 1 out]
              n136 = call "Request to Guardian.vi"("Data"=FALSE, "Requests"=Requests."Run Stopped with Errors", "Father of all uServices in"=w436) -> ("Father of all uServices out"=w438:refnum<class "Tamer.lvclass">)  [unwired: 7 in, 1 out]
            }
          }
        }
        frame "Timeout of RUN" {
          # "Checks if someone has already stopped Timeout of RUN (but this message has already get enqueued): in case, do nothing, because it means that the RUN Init Procedure has completed successfully (albeit just in time). In case Timeout of RUN was still on, terminate the RUN Init Procedure and thow the timeout error."
          # "Stop the RUN Init Procedure and raise ABORT."
          n137 = call-dynamic "Infinite Message Manager.vi"("Father of all uServices in"=w469, "Consumer Case Selector"=Tamer_Consumer_Case_Selector."Timeout of RUN" ("Monkey Consumer Case Selector"), "Infinite Message Selector"=Infinite_Message_Selector."Check") -> ("Father of all uServices out"=w473:refnum<class "Tamer.lvclass">, "Exists?"=w472:bool, "error out"=w471:errorcluster)  [unwired: 10 in]
          n138 = case shown="True" w472 {
            tunnel: [w476 w482] -> w466
            tunnel: w473 -> [w476 w477]
            tunnel: [w475 w481] -> w474
            tunnel: w471 -> [w475 w479]
            frame False {
            }
            frame True {
              # "#5778"
              n139 = call "Substitute Error.vi"("LabVIEW Object"=w477, "error in (no error)"=w479, "Error Code"=5778) -> ("error out"=w478:errorcluster)  [unwired: 8 in]
              n140 = call "Stop Initiate RUN Procedure.vi"("error in (no error)"=w478, "Tamer in"=w477) -> ("error out"=w481:errorcluster, "Tamer out"=w482:refnum<class "Tamer.lvclass">)  [unwired: 8 in]
            }
          }
          n141 = Merge Errors(w474, w468) -> (w467:errorcluster)
        }
        frame "Update from Monkey" {
          n142 = Variant To Data(error in=w488, type=T17 {"Monkey ID"="", "Monkey Status"=enum."Init", "Scripts left"=0, "ETA"="", "Current Action"="", "Report from previous RUNs"="", "Skipped RUNs"=refnum} ("Monkey Status Message"), Variant=w490) -> (data=w483:T17, error out=w484:errorcluster)
          n143 = case shown="No Error" w484 {
            selector: w484 -> [w500 w550]
            tunnel: [w493 w548] -> w487
            tunnel: [w492 w549] -> w486
            tunnel: w485 -> [w501 w548]
            tunnel: w483 -> [w499 _]
            frame No Error {
              n144 = Unbundle By Name(w499) -> ("Monkey ID"=w496:string, "Monkey Status"=w491:T18)
              n145 = call-dynamic "Process Monkey Report.vi"("error in (no error)"=w500, "Monkey Status Message"=w499, "Tamer in"=w501) -> ("error out"=w504:errorcluster, "Tamer out"=w505:refnum<class "Tamer.lvclass">)  [unwired: 7 in]
              n146 = Concatenate Strings("Received update from " ("string"), w496) -> (w498:string)
              n147 = call-dynamic "Update Action History.vi"("error in (no error)"=w504, "Action"=w498, "Tamer in"=w505) -> ("error out"=w502:errorcluster, "Tamer out"=w503:refnum<class "Tamer.lvclass">)  [unwired: 7 in]
              n148 = call-dynamic "Get Status of Monkeys.vi"("error in (no error)"=w502, "Tamer in"=w503) -> ("error out"=w506:errorcluster, "Anything running?"=w508:bool, "Tamer out"=w507:refnum<class "Tamer.lvclass">)  [unwired: 7 in]
              n149 = case shown="False" w508 {
                tunnel: w507 -> [w528 w541]
                tunnel: w506 -> [w527 w543]
                tunnel: [w518 w544] -> w495
                tunnel: [w517 w542] -> w494
                tunnel: w496 -> [w526 _]
                frame False {
                  n150 = Unbundle By Name(w528) -> ("STOPPED"=w529:bool)
                  n151 = case shown="True" w529 {
                    tunnel: w528 -> [w533 w540]
                    tunnel: w527 -> [w532 w539]
                    tunnel: [w533 w540] -> w523
                    tunnel: [w532 w539] -> w520
                    tunnel: w526 -> [_ w535]
                    tunnel: [w530 w534] -> w519
                    frame False {
                      w530 = "All Monkeys Finished" ("Action")
                      n152 = call "Temporised Pop-up Window.vi"("error in (no error)"=w532, "Timeout"=5.0, "Text"=w530) -> ()  [unwired: 8 in, 1 out]
                    }
                    frame True {
                      n153 = call <vilib>:"Space Constant.vi"() -> ("String"=w538:string)
                      n154 = Concatenate Strings("STOPPED:" ("string"), w535, w538, " Finished" ("Action")) -> (w534:string)
                    }
                  }
                  n155 = call "Request to Guardian.vi"("error in (no error)"=w520, "Data"=FALSE, "Requests"=Requests."Update Run Status", "Father of all uServices in"=w523) -> ("error out"=w521:errorcluster, "Father of all uServices out"=w522:refnum<class "Tamer.lvclass">)  [unwired: 6 in]
                  n156 = call-dynamic "Update Action History.vi"("error in (no error)"=w521, "Action"=w519, "Tamer in"=w522) -> ("error out"=w517:errorcluster, "Tamer out"=w518:refnum<class "Tamer.lvclass">)  [unwired: 7 in]
                }
                frame True {
                  n157 = call "Request to Guardian.vi"("error in (no error)"=w543, "Data"=TRUE, "Requests"=Requests."Update Run Status", "Father of all uServices in"=w541) -> ("error out"=w542:errorcluster, "Father of all uServices out"=w544:refnum<class "Tamer.lvclass">)  [unwired: 6 in]
                }
              }
              n158 = case shown="\"Finished (with errors)\"" w491 {
                tunnel: w495 -> [w510 w514]
                tunnel: w494 -> [w509 w513]
                tunnel: [w510 w512] -> w493
                tunnel: [w509 w511] -> w492
                frame Default {
                }
                frame "Finished (with errors)" {
                  n159 = call "Request to Guardian.vi"("error in (no error)"=w513, "Data"=FALSE, "Requests"=Requests."Run Stopped with Errors", "Father of all uServices in"=w514) -> ("error out"=w511:errorcluster, "Father of all uServices out"=w512:refnum<class "Tamer.lvclass">)  [unwired: 6 in]
                }
              }
            }
            frame Error {
              # "#5207"
              n160 = call "Substitute Error.vi"("LabVIEW Object"=w548, "error in (no error)"=w550, "Error Code"=5207) -> ("error out"=w549:errorcluster)  [unwired: 8 in]
            }
          }
        }
        frame "Monkey Died" {
          n161 = Variant To Data(error in=w556, type="" ("Monkey ID"), Variant=w558) -> (data=w554:string, error out=w555:errorcluster)
          n162 = case shown="No Error" w555 {
            selector: w555 -> [w570 w587]
            tunnel: w554 -> [w567 _]
            tunnel: w553 -> [w576 w588]
            tunnel: [w559 w588] -> w552
            tunnel: [w560 w586] -> w551
            frame No Error {
              w564 = "The Stage" ("FP Item Name")
              n163 = call-poly "Get GUI Item Value.vi"("FP Item Name"=w564, "uService Template in"=w576) -> ("error out"=w575:errorcluster, "Value"=w574:variant)  [unwired: 7 in, 1 out]
              n164 = Unbundle By Name(w576) -> ("Monkeys"=w572:map{string, string[]})
              n165 = Variant To Data(error in=w575, type=T19[][] [] ("2D Synchronous Monkeys"), Variant=w574) -> (data=w569:T19[][])  [unwired: 1 out]
              n166 = Collection Size(1:w572) -> (0:w571:i32)
              n167 = call "Cast 2D to 1D.vi"("1D size"=w571, "2D Synchronous Monkeys"=w569) -> ("1D Synchronous Monkeys"=w568:T19[])
              n168 = call-dynamic "Monkey Died.vi"("error in (no error)"=w570, "Monkey ID"=w567, "Tamer in"=w576) -> ("error out"=w562:errorcluster, "Tamer out"=w563:refnum<class "Tamer.lvclass">)  [unwired: 7 in]
              n169 = for {
                tunnel: w568 -> [w584] mode=indexing
                tunnel: w567 -> [w583]
                tunnel: [w584] -> w566 mode=indexing if=w578
                # "Remove the Monkey from the GUI"
                n170 = Unbundle By Name(w584) -> ("Monkey ID"=w582:string)
                n171 = Empty String/Path?(string/path=w582) -> (empty?=w581:bool)
                n172 = Not Equal?(x=w582, y=w583) -> (x != y?=w579:bool)
                n173 = Not(x=w581) -> (.not. x?=w580:bool)
                n174 = And(x=w580, y=w579) -> (x .and. y?=w578:bool)
              }
              n175 = call-dynamic "Update Process Indicator.vi"("error in (no error)"=w562, "Tamer in"=w563) -> ("error out"=w561:errorcluster, "Tamer out"=w577:refnum<class "Tamer.lvclass">)  [unwired: 8 in]
              n176 = call "Cast 1D to 2D.vi"("1D Monkeys"=w566) -> ("2D Monkeys"=w565:T19[][])
              n177 = call "Update GUI.vi"("error in (no error)"=w561, "Data"=w565, "GUI Item Name"=w564, "uService Template in"=w577) -> ("error out"=w560:errorcluster, "uService Template out"=w559:refnum<class "Tamer.lvclass">)  [unwired: 6 in]
            }
            frame Error {
              # "#5773"
              n178 = call "Substitute Error.vi"("LabVIEW Object"=w588, "error in (no error)"=w587, "Error Code"=5773) -> ("error out"=w586:errorcluster)  [unwired: 8 in]
            }
          }
        }
        frame "Reschedule" {
          w598 = ""  # Process ID
          # "#5775"
          n179 = Variant To Data(error in=w600, type=w598, Variant=w599) -> (data=w589:string, error out=w597:errorcluster)
          n180 = case shown="\"ALL\"" w589 {
            selector: w589 -> [_ w618]
            tunnel: w593 -> [w616 w622]
            tunnel: w597 -> [w614 w621]
            tunnel: [w616 w620] -> w601
            tunnel: [w615 w617] -> w603
            tunnel: [w614 w619] -> w602
            frame "ALL" {
              n181 = Unbundle By Name(w616) -> ("Schedules"=w615:refnum<class "Schedule.lvclass">[])  [unwired: 1 out]
            }
            frame Default {
              n182 = call-dynamic "Get Schedules for the Process.vi"("error in (no error)"=w621, "Process ID"=w618, "Tamer in"=w622) -> ("error out"=w619:errorcluster, "Schedules"=w617:refnum<class "Schedule.lvclass">[], "Tamer out"=w620:refnum<class "Tamer.lvclass">)  [unwired: 5 in, 1 out]
            }
          }
          n183 = call "Message to uService.vi"("Father of all uServices in"=w601, "uService ID"="Scheduler" ("string"), "Message"="Reschedule", "Data"=w603, "error in (no error)"=w602) -> ("Father of all uServices out"=w592:refnum<class "Tamer.lvclass">, "error out"=w590:errorcluster)  [unwired: 9 in]
          n184 = call-dynamic "Get List of Monkeys in the Process.vi"("error in (no error)"=w590, "Process ID"=w589, "Tamer in"=w592) -> ("error out"=w613:errorcluster, "List of Monkeys"=w596:string[], "Tamer out"=w591:refnum<class "Tamer.lvclass">)  [unwired: 5 in, 1 out]
          n185 = call <vilib>:"Space Constant.vi"() -> ("String"=w608:string)
          n186 = call <vilib>:"1D String Array to Delimited String.vi"("delimiter"=", ", "string array"=w596) -> ("delimited string"=w594:string)  [unwired: 9 in]
          n187 = Concatenate Strings("Sending the schedule(s) from" ("string"), w608, w594) -> (w607:string)
          n188 = call-dynamic "Update Action History.vi"("error in (no error)"=w613, "Action"=w607, "Tamer in"=w591) -> ("error out"=w610:errorcluster, "Tamer out"=w612:refnum<class "Tamer.lvclass">)  [unwired: 7 in]
          n189 = call "Substitute Error.vi"("LabVIEW Object"=w612, "error in (no error)"=w610, "Error Code"=5775, "Optional String"=w594) -> ("error out"=w611:errorcluster)  [unwired: 7 in]
        }
        frame "Rerun" {
          w630 = ""  # Process ID
          # "#5774"
          n190 = Variant To Data(error in=w631, type=w630, Variant=w632) -> (data=w626:string, error out=w629:errorcluster)
          n191 = call-dynamic "Get Status of Monkeys.vi"("Tamer in"=w628) -> ("Anything running?"=w624:bool, "Tamer out"=w627:refnum<class "Tamer.lvclass">)  [unwired: 8 in, 1 out]
          n192 = Empty String/Path?(string/path=w626) -> (empty?=w625:bool)
          n193 = Or(x=w624, y=w625) -> (x .or. y?=w623:bool)
          n194 = case shown="False" w623 {
            tunnel: [w641 w676] -> w634
            tunnel: [w640 w675] -> w633
            tunnel: w629 -> [w639 w675]
            tunnel: w627 -> [w638 w676]
            tunnel: w626 -> [w637 _]
            frame False {
              n195 = case "Update Monkey status" shown="\"ALL\"" w637 {
                selector: w637 -> [w644 _]
                tunnel: [w653 w671] -> w641
                tunnel: [w651 w670] -> w640
                tunnel: w639 -> [w642 w667]
                tunnel: w638 -> [w643 w664]
                frame Default {
                  # "Update status of Monkeys in the proces"
                  n196 = call-dynamic "Get Schedules for the Process.vi"("error in (no error)"=w642, "Process ID"=w644, "Tamer in"=w643) -> ("error out"=w647:errorcluster, "Schedules"=w646:refnum<class "Schedule.lvclass">[], "Sync. Mask"=w645:T3[], "Tamer out"=w648:refnum<class "Tamer.lvclass">)  [unwired: 5 in]
                  n197 = call "Send Schedules to Monkeys.vi"("error in (no error)"=w647, "Schedules"=w646, "Sync. Mask"=w645, "Tamer in"=w648) -> ("error out"=w649:errorcluster, "Tamer out"=w650:refnum<class "Tamer.lvclass">)  [unwired: 6 in]
                  n198 = call-dynamic "Get List of Monkeys in the Process.vi"("error in (no error)"=w649, "Process ID"=w644, "Tamer in"=w650) -> ("error out"=w654:errorcluster, "List of Monkeys"=w655:string[], "Tamer out"=w656:refnum<class "Tamer.lvclass">)  [unwired: 5 in, 1 out]
                  n199 = for {
                    tunnel: w655 -> [w660] mode=indexing
                    tunnel: w654 -> [w661]
                    shift-right: [w659] -> w653
                    shift-left: w656 -> [w662]
                    tunnel: [w658] -> w652 mode=indexing
                    n200 = call-dynamic "Update Monkeys Status.vi"("Overwrite"=TRUE, "error in (no error)"=w661, "Status"=Monkey_Status."Init", "Monkey ID"=w660, "Tamer in"=w662) -> ("error out"=w658:errorcluster, "Tamer out"=w659:refnum<class "Tamer.lvclass">)  [unwired: 5 in]
                  }
                  n201 = Merge Errors(w652) -> (w651:errorcluster)
                }
                frame "ALL" {
                  # "Update status of all the Monkeys"
                  n202 = Unbundle By Name(w664) -> ("Sync. Mask"=w665:T3[], "Schedules"=w666:refnum<class "Schedule.lvclass">[])
                  n203 = call "Send Schedules to Monkeys.vi"("error in (no error)"=w667, "Schedules"=w666, "Sync. Mask"=w665, "Tamer in"=w664) -> ("error out"=w674:errorcluster, "Tamer out"=w668:refnum<class "Tamer.lvclass">)  [unwired: 6 in]
                  n204 = call-dynamic "Update Monkeys Status.vi"("Overwrite"=TRUE, "In ALL?"=TRUE, "error in (no error)"=w674, "Status"=Monkey_Status."Init", "Tamer in"=w668) -> ("error out"=w670:errorcluster, "Tamer out"=w671:refnum<class "Tamer.lvclass">)  [unwired: 5 in]
                }
              }
            }
            frame True {
            }
          }
          n205 = call "Substitute Error.vi"("LabVIEW Object"=w634, "error in (no error)"=w633, "Error Code"=5774) -> ("error out"=w636:errorcluster)  [unwired: 8 in]
        }
        frame "Stop Schedule" {
          w686 = T14 {"Gracefully"=FALSE, "Process"="ALL"} ("cluster")
          # "Check if the process is parallel and the gracefully flag is False, turn off the DAQ and request the STOP RUN"
          # "Just send stop schedule to Monkey with the gracefully flag"
          # "This is pretty much the new Stop Run"
          # "Stop the schedule"
          n206 = call-dynamic "Stop Periodic Replies Checks.vi"("Tamer in"=w677) -> ("Tamer out"=w678:refnum<class "Tamer.lvclass">)  [unwired: 9 in, 1 out]
          n207 = Variant To Data(type=w686, Variant=w682) -> (data=w687:T14, error out=w685:errorcluster)  [unwired: 1 in]
          n208 = property class="Tamer.lvclass"(reference=w678) -> (reference out=w688:refnum<class "Tamer.lvclass">, "Accessors:STOPPED"=w684:bool)  [unwired: 1 in, 1 out]
          n209 = case shown="Error .." w685 {
            tunnel: ["Stop button pressed. Sending STOP!" ("initial string") "Error occurred, sending STOP! " ("initial string")] -> w679
            frame No Error {
            }
            frame Error {
            }
          }
          n210 = Select(t=w686, s=w685, f=w687) -> (s? t:f=w683:T14)
          n211 = case shown="False" w684 {
            tunnel: w688 -> [w697 w748]
            tunnel: [w706 w748] -> w681
            tunnel: [w705 errorcluster {"status"=FALSE, "code"=0, "source"=""} ("error out")] -> w680
            tunnel: w683 -> [w704 _]
            tunnel: w679 -> [w695 _]
            frame False {
              # "Here it should send stop to whatever is still running. No point of sending to all"
              # "The schedules were not stopped yet"
              n212 = call-dynamic "Update Action History.vi"("Action"=w695, "Tamer in"=w697) -> ("Tamer out"=w696:refnum<class "Tamer.lvclass">)  [unwired: 8 in, 1 out]
              n213 = Unbundle By Name(w704) -> ("Process"=w699:string, "Gracefully"=w703:bool)
              n214 = Unbundle By Name(w696) -> ("Sync. Mask"=w693:T3[], "Sync. Process ID"=w702:string)
              n215 = Equal?(x=w702, y=w699) -> (x = y?=w691:bool)
              n216 = Equal?(x=w699, y="ALL") -> (x = y?=w692:bool)
              n217 = Empty Array?(array=w693) -> (empty?=w690:bool)
              n218 = Compound Arithmetic op=OR(w690, w691, w692) -> (w689:bool)
              n219 = case shown="False" w689 {
                selector: w689 -> [w713 w715]
                tunnel: w696 -> [w712 w714]
                tunnel: [w712 w718] -> w700
                tunnel: [errorcluster {"status"=FALSE, "code"=0, "source"=""} ("error out") w716] -> w710
                tunnel: [w713 w715] -> w698
                frame False {
                  # "Single process"
                }
                frame True {
                  # "Update stop flag"
                  n220 = call-dynamic "Write STOPPED.vi"("STOPPED"=TRUE, "Monkey in"=w714) -> ("error out"=w716:errorcluster, "Monkey out"=w718:refnum<class "Tamer.lvclass">)  [unwired: 8 in]
                }
              }
              n221 = case shown="False" w703 {
                tunnel: w700 -> [w723 w746]
                tunnel: [w721 w746] -> w709
                tunnel: w710 -> [w722 w745]
                tunnel: [w720 w745] -> w708
                tunnel: [_ TRUE] -> w694
                tunnel: w698 -> [w719 _]
                frame False {
                  # "Not gracefully. If stop is issued for all processes or synchronised process we need to handle the request of StopRun and the DAQ"
                  n222 = case shown="True" w719 {
                    tunnel: w723 -> [w725 w726]
                    tunnel: w722 -> [w724 w727]
                    tunnel: [w725 w729] -> w721
                    tunnel: [w724 w728] -> w720
                    frame False {
                    }
                    frame True {
                      # "#STOP_DAQ"
                      n223 = in-place {
                        in-place-border: w727 -> [w736]
                        in-place-border: [w735] -> w733
                        in-place-border: w726 -> [w734]
                        # "request the StopRun"
                        n224 = in-place-cluster #2(w726) -> ("StartRun/StopRun toggle"=w737:bool)
                        n225 = case shown="False" w737 {
                          tunnel: w736 -> [w739 w742]
                          tunnel: [w739 w741] -> w735
                          tunnel: w734 -> [_ w743]
                          frame False {
                          }
                          frame True {
                            # "#STOP_RUN"
                            n226 = call "Request to Guardian.vi"("error in (no error)"=w742, "Requests"=Requests."Stop RUN", "Father of all uServices in"=w743) -> ("error out"=w741:errorcluster)  [unwired: 7 in, 1 out]
                          }
                        }
                        n227 = in-place-cluster #2("StartRun/StopRun toggle"=FALSE) -> (w732:refnum<class "Tamer.lvclass">)
                      }
                      n228 = call "Message to uService.vi"("Father of all uServices in"=w732, "uService ID"="DAQ Manager", "Message"="Stop Run", "error in (no error)"=w733) -> ("Father of all uServices out"=w729:refnum<class "Tamer.lvclass">, "error out"=w728:errorcluster)  [unwired: 10 in]
                    }
                  }
                }
                frame True {
                  # "In gracefull stop we don't have to do anything. The script will return banana and the standard operation will proceed"
                }
              }
              n229 = call-dynamic "Message to All Monkeys in the Process.vi"("Tamer in"=w709, "Process ID"=w699, "Message"="Stop Schedule", "Data"=w694, "error in (no error)"=w708) -> ("Tamer out"=w706:refnum<class "Tamer.lvclass">, "error out"=w705:errorcluster)  [unwired: 9 in]
            }
            frame True {
              # "Stopped already"
            }
          }
        }
        frame "Skip Run" {
          n230 = call-dynamic "Read STOPPED.vi"("Monkey in"=w753) -> ("STOPPED"=w751:bool, "Monkey out"=w752:refnum<class "Tamer.lvclass">)  [unwired: 8 in, 1 out]
          n231 = case shown="False" w751 {
            tunnel: w757 -> [w772 w808]
            tunnel: w756 -> [w771 _]
            tunnel: w752 -> [w764 w809]
            tunnel: [w763 w809] -> w755
            tunnel: [w762 w808] -> w754
            frame False {
              w768 = T14 {"Gracefully"=FALSE, "Process"="ALL"} ("cluster")
              # "Nothing was stopped, we can send skip"
              n232 = Variant To Data(type=w768, Variant=w771) -> (data=w769:T14, error out=w770:errorcluster)  [unwired: 1 in]
              n233 = Select(t=w768, s=w770, f=w769) -> (s? t:f=w767:T14)
              n234 = Unbundle By Name(w767) -> ("Process"=w759:string, "Gracefully"=w761:bool)
              n235 = case shown="False" w761 {
                tunnel: w764 -> [w778 w807]
                tunnel: [w780 w807] -> w766
                tunnel: w772 -> [w781 w806]
                tunnel: [w779 w806] -> w765
                tunnel: w759 -> [w783 _]
                tunnel: [_ TRUE] -> w758
                frame False {
                  # "Not gracefully. If stop is issued for all processes or synchronised process we need to handle the request of StopRun and the DAQ"
                  n236 = Unbundle By Name(w778) -> ("Sync. Mask"=w774:T3[], "Sync. Process ID"=w784:string)
                  n237 = Empty Array?(array=w774) -> (empty?=w775:bool)
                  n238 = Equal?(x=w784, y=w783) -> (x = y?=w776:bool)
                  n239 = Equal?(x=w783, y="ALL") -> (x = y?=w777:bool)
                  n240 = Compound Arithmetic op=OR(w775, w776, w777) -> (w773:bool)
                  n241 = case shown="True" w773 {
                    tunnel: w778 -> [w786 w787]
                    tunnel: w781 -> [w785 w788]
                    tunnel: [w786 w790] -> w780
                    tunnel: [w785 w789] -> w779
                    frame False {
                    }
                    frame True {
                      # "#STOP_DAQ"
                      n242 = in-place {
                        in-place-border: w788 -> [w797]
                        in-place-border: [w796] -> w794
                        in-place-border: w787 -> [w795]
                        # "request the StopRun"
                        n243 = in-place-cluster #3(w787) -> ("StartRun/StopRun toggle"=w798:bool)
                        n244 = case shown="True" w798 {
                          tunnel: w797 -> [w800 w803]
                          tunnel: [w800 w802] -> w796
                          tunnel: w795 -> [_ w804]
                          frame False {
                          }
                          frame True {
                            # "#STOP_RUN"
                            n245 = call "Request to Guardian.vi"("error in (no error)"=w803, "Requests"=Requests."Stop RUN", "Father of all uServices in"=w804) -> ("error out"=w802:errorcluster)  [unwired: 7 in, 1 out]
                          }
                        }
                        n246 = in-place-cluster #3("StartRun/StopRun toggle"=FALSE) -> (w793:refnum<class "Tamer.lvclass">)
                      }
                      n247 = call "Message to uService.vi"("Father of all uServices in"=w793, "uService ID"="DAQ Manager", "Message"="Stop Run", "error in (no error)"=w794) -> ("Father of all uServices out"=w790:refnum<class "Tamer.lvclass">, "error out"=w789:errorcluster)  [unwired: 10 in]
                    }
                  }
                }
                frame True {
                  # "In gracefull skip we don't have to do anything. The script will return banana and the standard operation will proceed"
                }
              }
              n248 = call-dynamic "Message to All Monkeys in the Process.vi"("Tamer in"=w766, "Process ID"=w759, "Message"="Skip run", "Data"=w758, "error in (no error)"=w765) -> ("Tamer out"=w763:refnum<class "Tamer.lvclass">, "error out"=w762:errorcluster)  [unwired: 9 in]
            }
            frame True {
              # "Stopped, we don't have to do anything"
            }
          }
        }
        frame "Kill Process" {
          w811 = "ALL"
          n249 = Variant To Data(type=w811, Variant=w813) -> (data=w812:string, error out=w818:errorcluster)  [unwired: 1 in]
          n250 = Select(t=w811, s=w818, f=w812) -> (s? t:f=w810:string)
          n251 = call-dynamic "Kill Process.vi"("error in (no error)"=w816, "Process ID"=w810, "Tamer in"=w817) -> ("error out"=w815:errorcluster, "Tamer out"=w814:refnum<class "Tamer.lvclass">)  [unwired: 7 in]
        }
        frame "Update GV" {
          n252 = call "Generate Tamer Status.vi"("error in (no error)"=w822, "Monkey in"=w823) -> ("error out"=w819:errorcluster, "Tamer Panel"=w821:T21, "Monkey out"=w820:refnum<class "Tamer.lvclass">)  [unwired: 7 in]
          n253 = case shown="No Error" w819 {
            tunnel: w821 -> [w824 _]
            frame No Error {
              n254 = global write "Tamer GV.vi" "Tamer Panel"(w824) -> ()
            }
            frame Error {
            }
          }
        }
      }
    }
    frame Error {
    }
  }
  n255 = call-parent "Consumer.vi"("error in (no error)"=w8, "Data"="Data", "Case ID"="Case ID", "uService Template in"=w7) -> ("error out"=w3:errorcluster, "uService Template out"=w4:refnum<class "Tamer.lvclass">)  [unwired: 6 in]
  n256 = call-dynamic "Debug Info Display.vi"("Tamer in"=w4, "error in (no error)"=w3) -> ("Tamer out"=→"Tamer out":refnum<class "Tamer.lvclass">, "error out"=→"error out":errorcluster)  [unwired: 12 in]
